vi "Display Module.vi"(7 "Callling VI":refnum<vi>) -> ()   [LabVIEW 2021]
uses:
  Display Module TypeDefs/IMAQ Z Scale Bar.ctl
  <vilib>/Utility/miscctls.llb/LVPointTypeDef.ctl
  <vilib>/vision/Image Controls.llb/IMAQ Image.ctl
  Hardware Configuration/Hardware Configuration Controls/Standard Action.ctl
  <vilib>/Utility/miscctls.llb/LVRectTypeDef.ctl
  <vilib>/event_ctls.llb/lveventtype.ctl
  Tools/TIFF Image Read and Write/ImageJ TIF Type Defs/TIF Write Image Information.ctl
  <vilib>/vision/NI_Vision_Development_Module.lvlib
panel:
  in  "Max":i32
  in  "Min":i32
  in  "lock scale":bool
  in  "Settings Menu":T1
  in  "Settings":bool
  in  "Refresh Rate (ms)":u32=30
  in  "Z Scale Channel 6":T2
  in  "Z Scale Channel 5":T2
  in  "Z Scale Channel 4":T2
  in  "Z Scale Channel 3":T2
  in  "Z Scale Channel 2":T2
  in  "Z Scale Channel 1":T2
  out "Messages":string
  in  "Max Left":bool
  in  "Max Right":bool
  in  "Add Display":bool
  in  "Remove Display":bool
  in  "Exit":bool
  out "Channel 6":T3(plugin-control)
  out "Channel 5":T3(plugin-control)
  out "Channel 4":T3(plugin-control)
  out "Channel 3":T3(plugin-control)
  out "Channel 2":T3(plugin-control)
  out "Channel 1":T3(plugin-control)
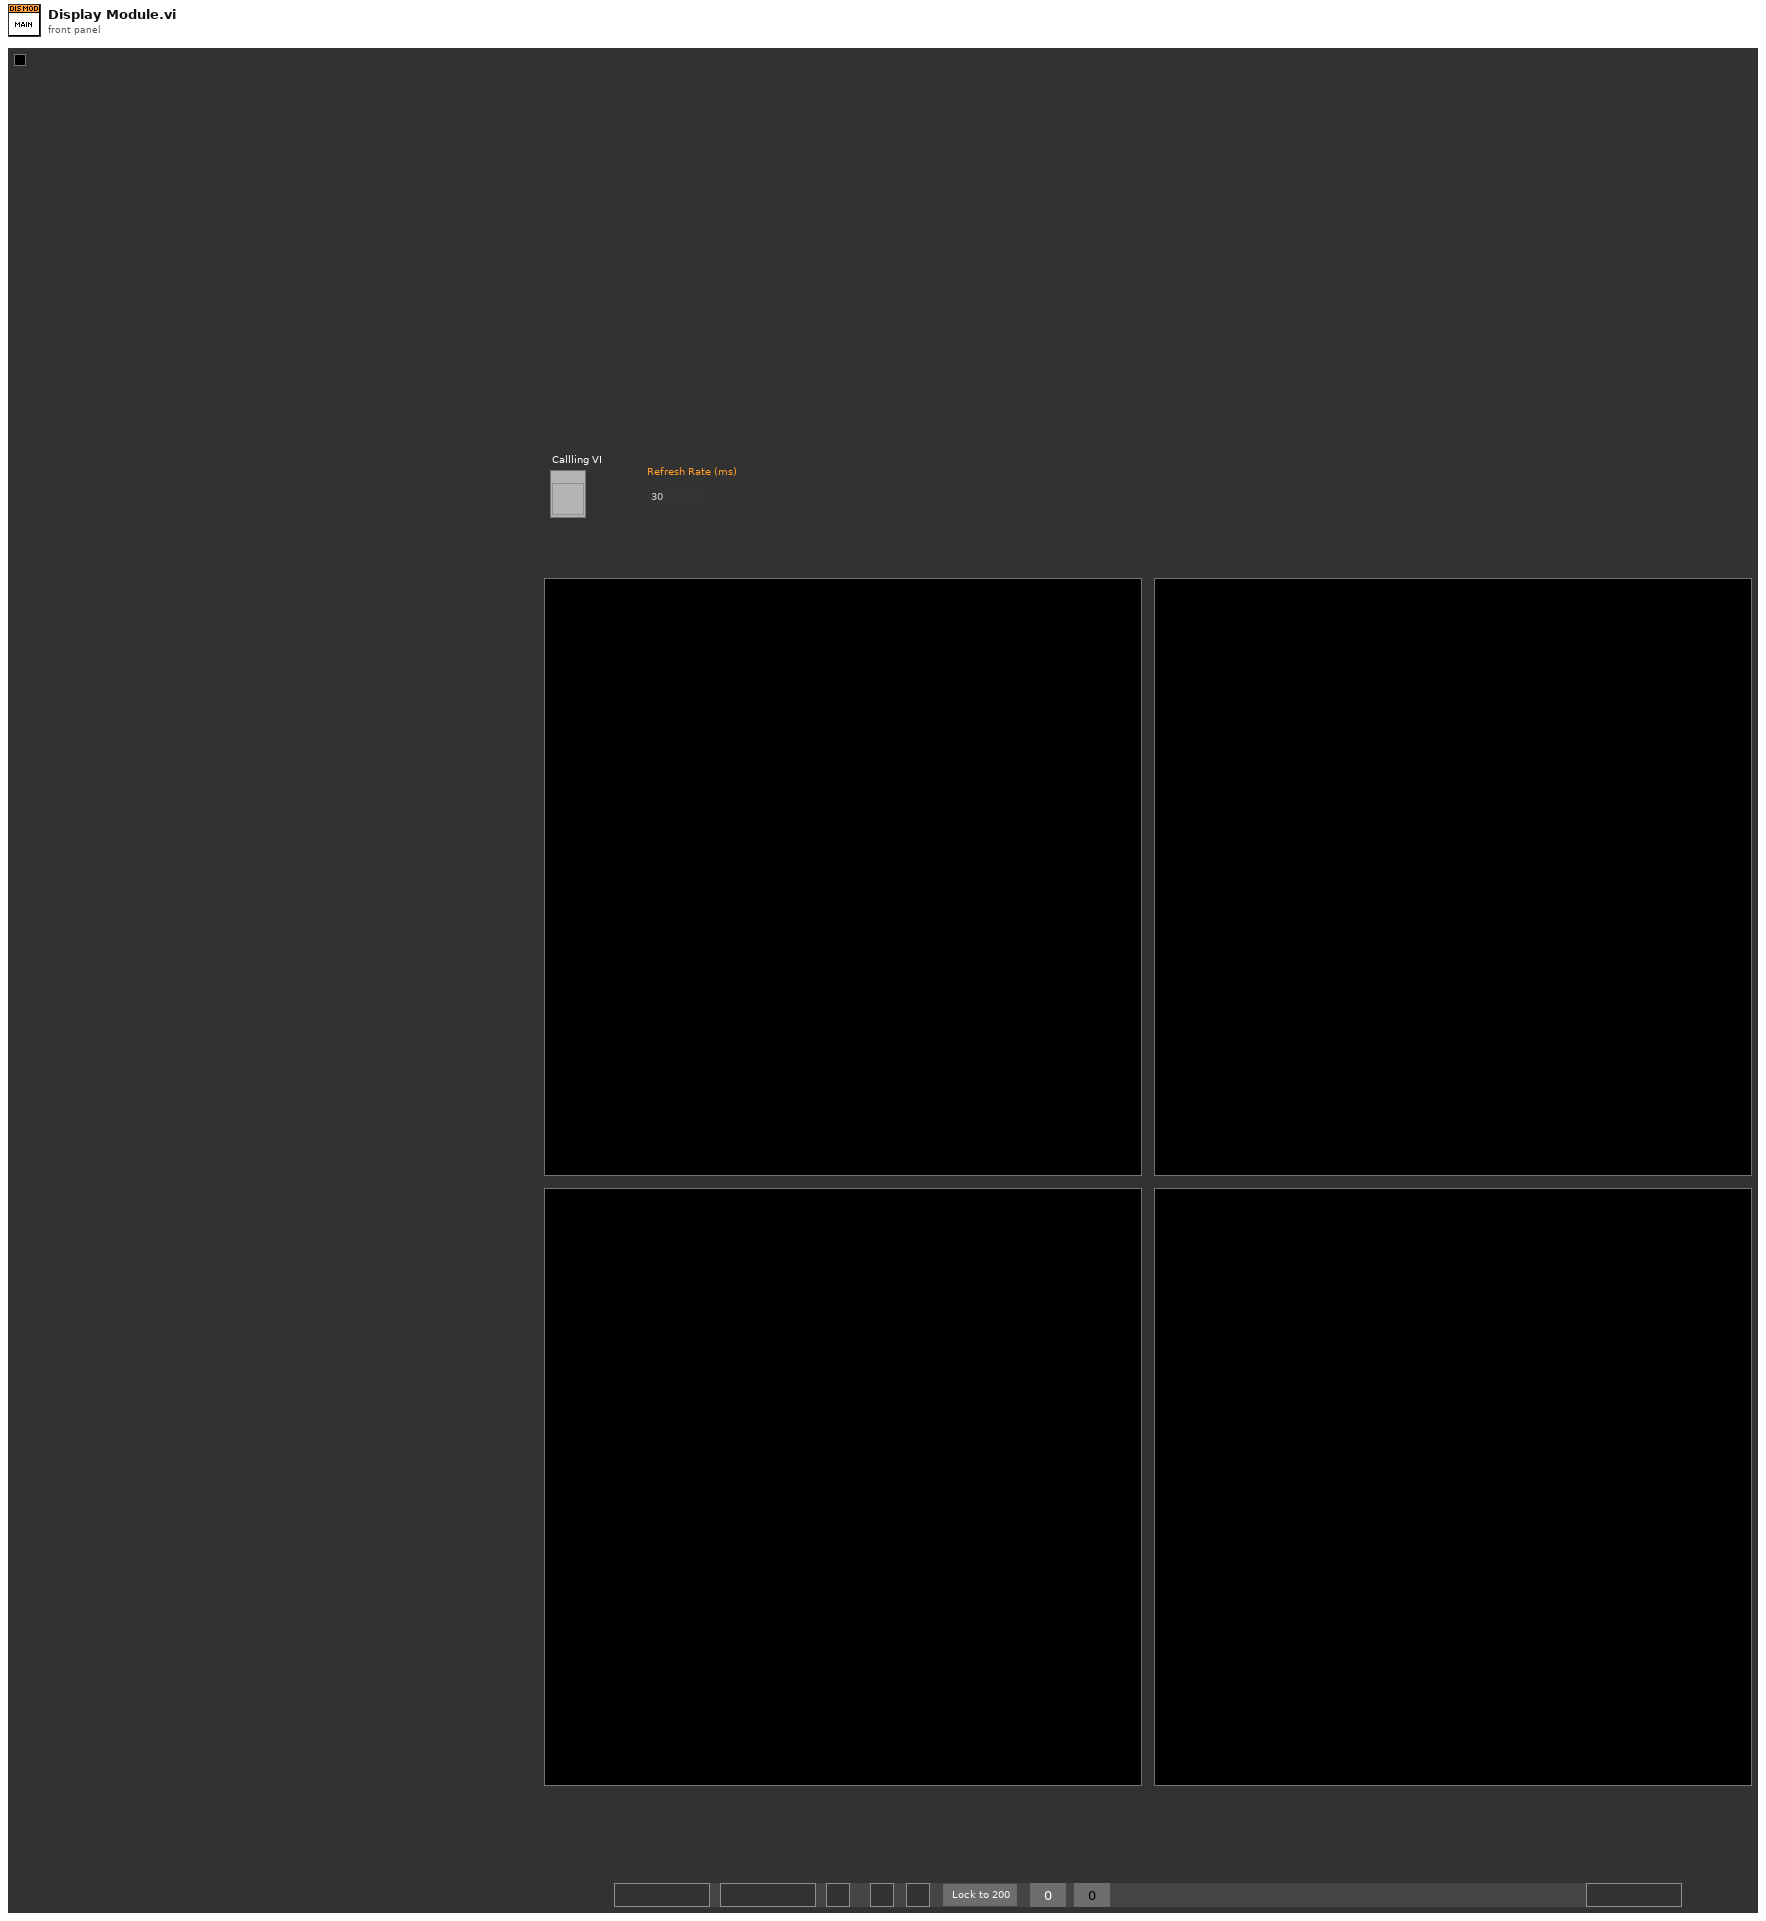
[diagram p1: front panel]
types:
  T1 = cluster{"Refresh Rate":bool, "Change Display Order":bool, "Display On / Off":bool}
  T2 = typedef "IMAQ Z Scale Bar.ctl" = cluster{"Z Scale Image":T3, "Z Scale Min":sgl, "Z Scale Max":sgl}
  T3 = typedef "IMAQ Image.ctl" = refnum<image>
  T4 = typedef "Standard Action.ctl" = enum16{"Read", "Write"}
  T5 = typedef "Image Type" = u32
  T6 = typedef "LVPointTypeDef.ctl" = cluster{"Horizontal":i16, "Vertical":i16}
  T7 = enum32{"Invalid", "Standard", "Closed", "Hidden", "Minimized", "Maximized"}
  T8 = enum16{"Always On", "Always Off", "Off While Running"}
  T9 = enum16{"Change Number", "Refresh Positions", "Get No. of Displays"}
  T10 = typedef "LVRectTypeDef.ctl" = cluster{"Left":i16, "Top":i16, "Right":i16, "Bottom":i16}
  T11 = typedef "lveventtype.ctl" = enum32{"Null", "Timeout", "Annotation Menu Selection", "Annotation Menu Selection?", "App Instance Close", "App Instance Close?", "Autoscale Range Change", "Bookmark Info Change", "Cell Edit", "Cell Edit?", "Cursor Grab", "Cursor Grab?", "Cursor Menu Selection", "Cursor Menu Selection?", "Cursor Move", "Cursor Release", "Data Change", "Direction Change", "Display State Change", "Drag Ended", "Drag Enter", "Drag Leave", "Drag Over", "Drag Source Update", "Drag Starting", "Drag Starting?", "Drop", "Exec State Change", "Key Down", "Key Down?", "Key Repeat", "Key Repeat?", "Key Up", "Listbox Double Click", "Menu Activation?", "Menu Selection (App)", "Menu Selection? (App)", "Menu Selection (User)", "Mouse Down", "Mouse Down?", "Mouse Enter", "Mouse Leave", "Mouse Move", "Mouse Up", "Mouse Wheel", "NI Security User Change (App)", "Pane Size", "Panel Close", "Panel Close?", "Panel Resize", "Plot Attribute Change", "Scale Range Change", "Shortcut Menu Activation?", "Shortcut Menu Selection (App)", "Shortcut Menu Selection? (App)", "Shortcut Menu Selection (User)", "Tree Double Click", "Tree Drag", "Tree Drag?", "Tree Drop", "Tree Drop?", "Tree Item Close", "Tree Item Close?", "Tree Item Open", "Tree Item Open?", "User Event", "Value Change"}
  T12 = cluster{"Global Rectangle":i32[], "Contours":cluster{"Contour Type":u32, "ROI Type":u32, "Points":i32[]}[]}
  T13 = cluster{"Mean Value":sgl, "Standard Variation":sgl, "Minimal Value":sgl, "Maximal Value":sgl, "Area (calibrated)":sgl, "Area (pixels)":u32, "%":sgl, "Calibration Valid":bool}
  T14 = typedef "TIF Write Image Information.ctl" = cluster{"Image Width (Pixels)":u32, "Image Height (Pixels)":u32, "Pixel Width (µm)":dbl, "Pixel Height (µm)":dbl, "Bits Per Sample (e.g. 16)":u32, "No. of Frames":u32, "No. of Slices":u32, "Time Step (sec)":dbl, "Z Step (µm)":dbl}
  T15 = typedef "LVAllMonitorsDisplayTypeDef.ctl" = cluster{"Bounds":cluster{"Left":i16, "Top":i16, "Right":i16, "Bottom":i16}, "Depth":i16}[]
  T16 = cluster{"Bounds":cluster{"Left":i16, "Top":i16, "Right":i16, "Bottom":i16}, "Depth":i16}
  T17 = enum16{"big-endian, network order", "native, host order", "little-endian"}
  T18 = cluster{"Contour Type":u32, "ROI Type":u32, "Points":i32[]}[]
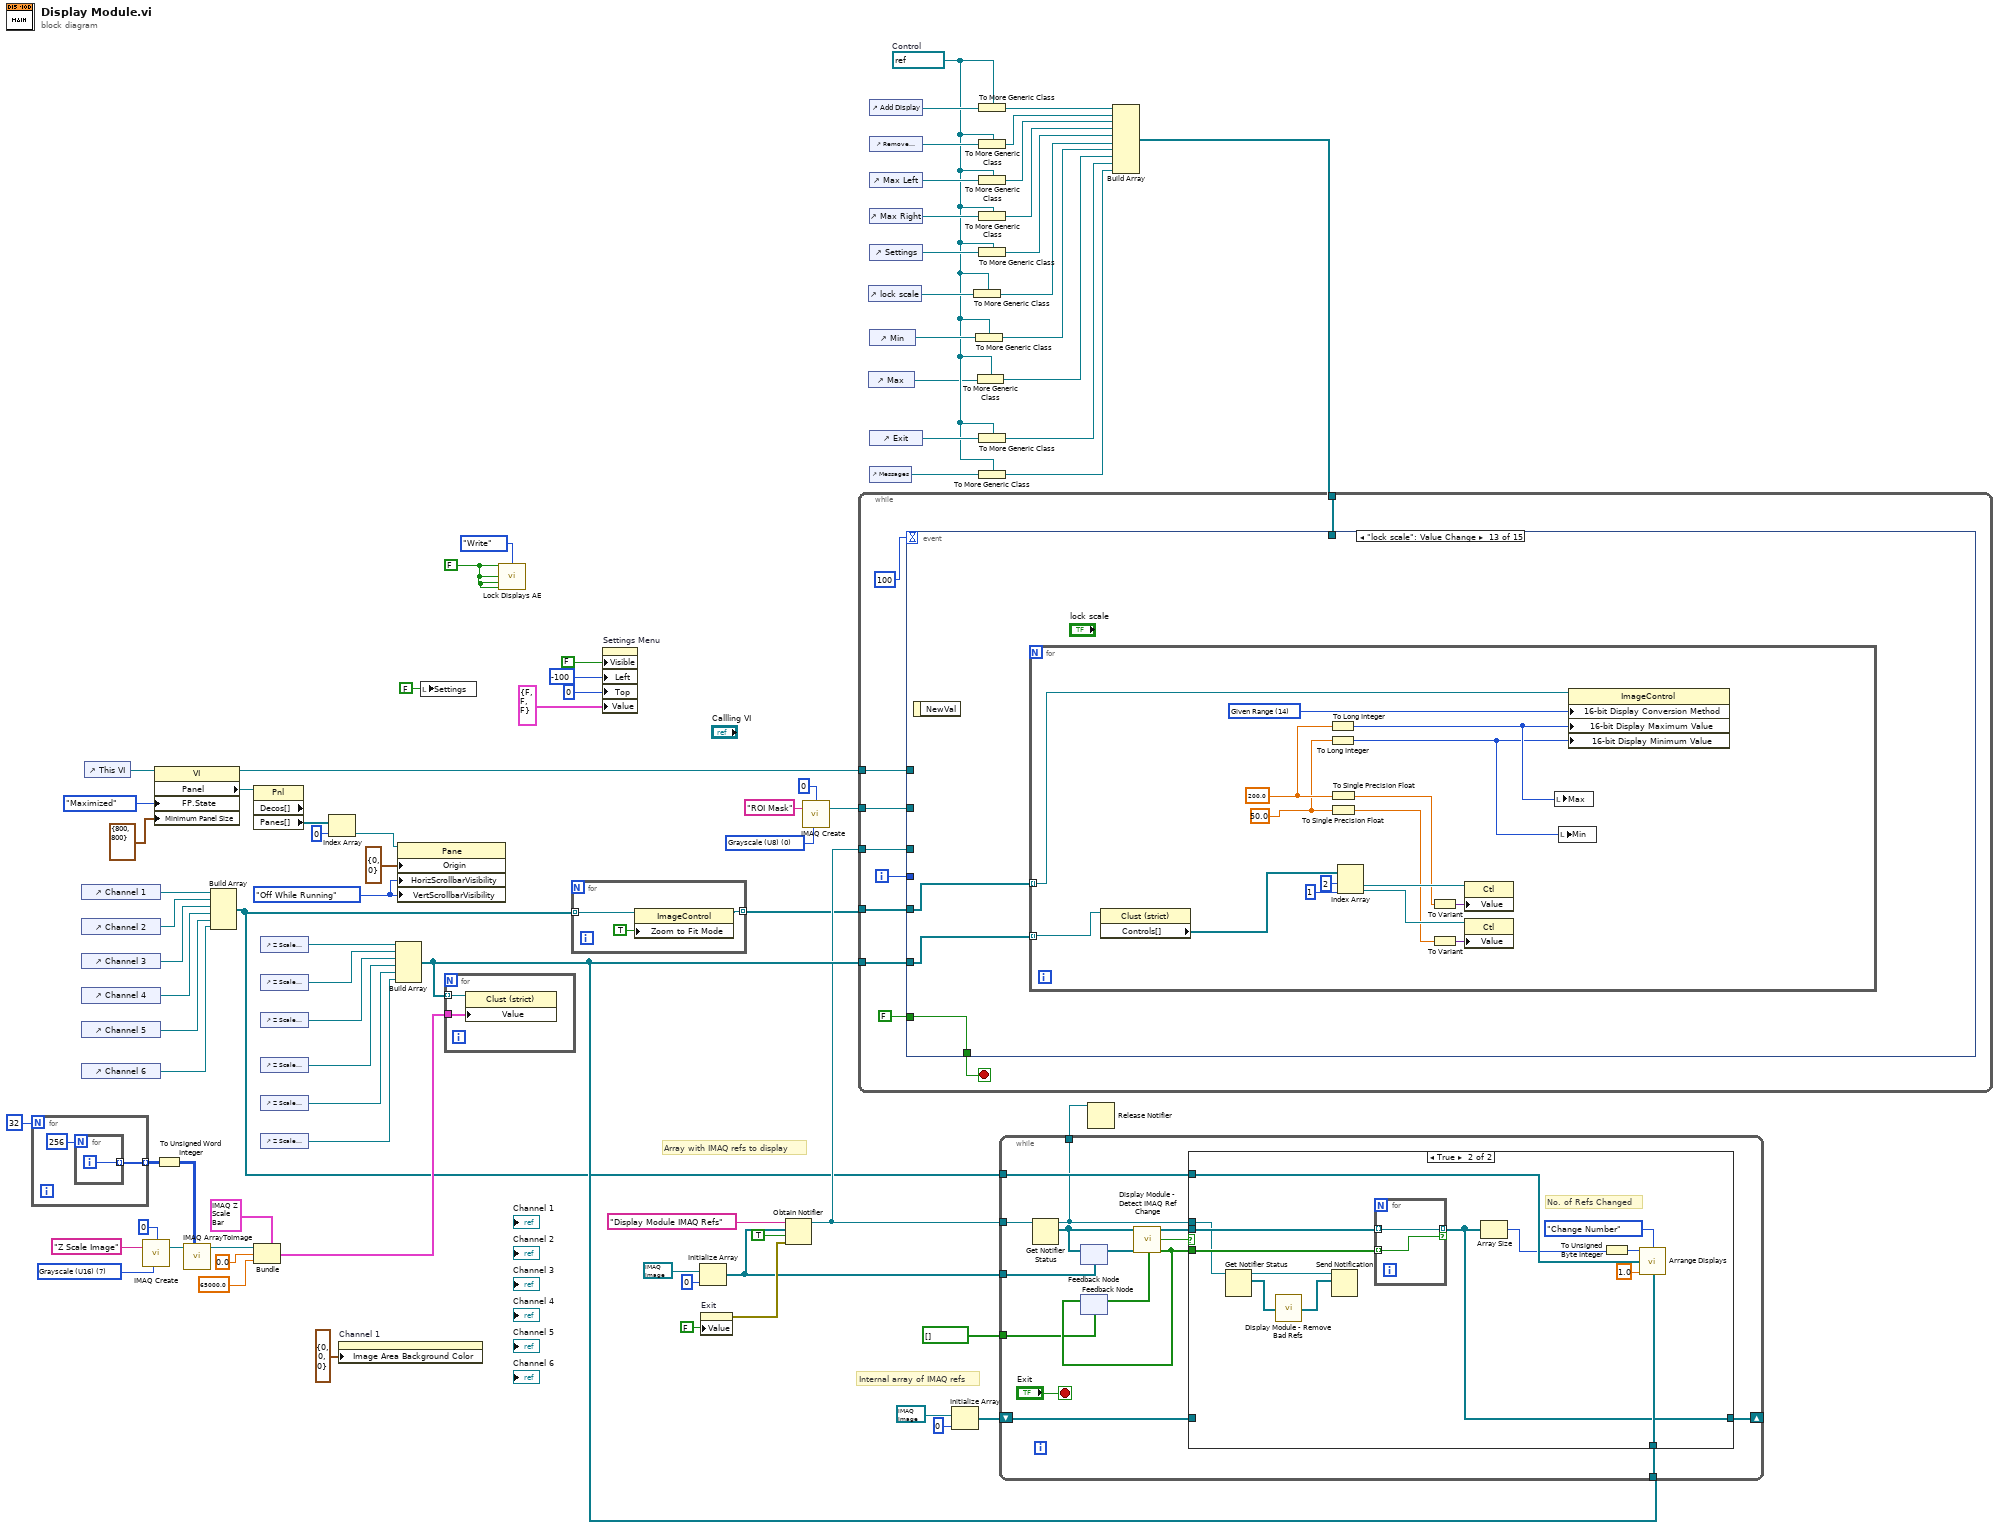
[diagram p0: block diagram]
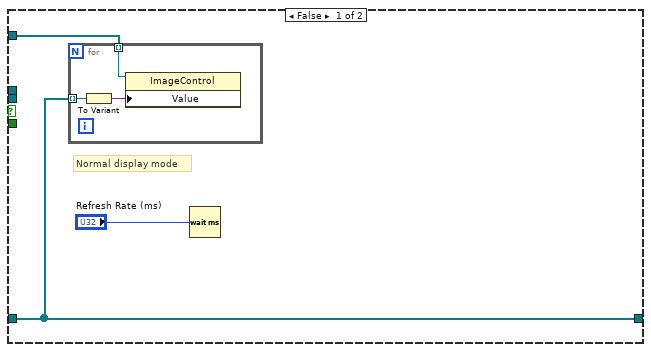
[diagram p2: hidden frame]
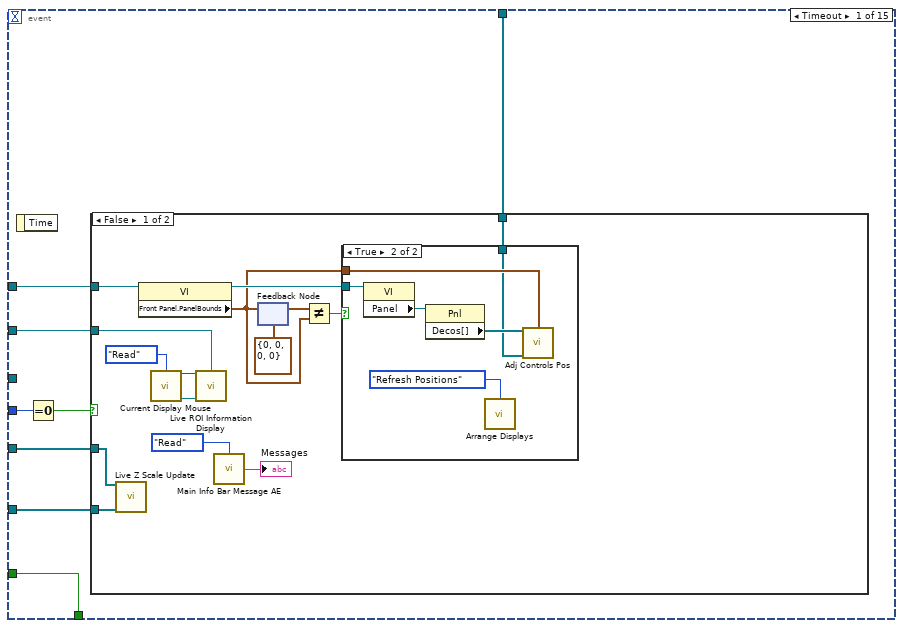
[diagram p3: hidden frame]
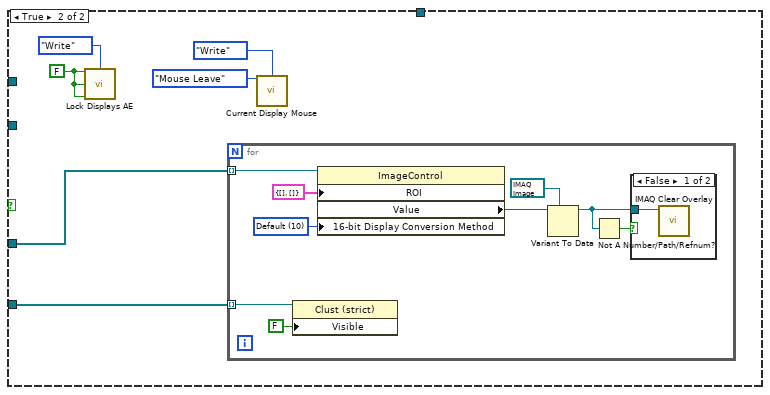
[diagram p5: hidden frame]
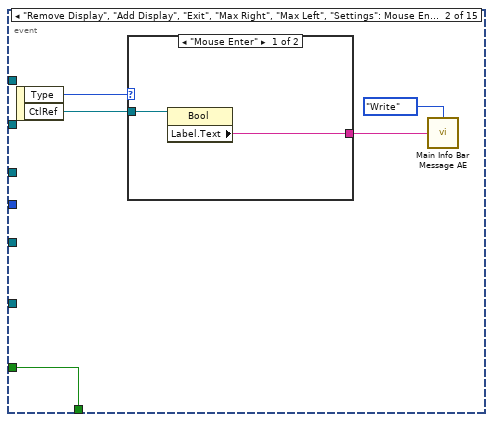
[diagram p7: hidden frame]
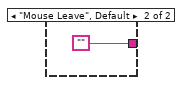
[diagram p8: hidden frame]
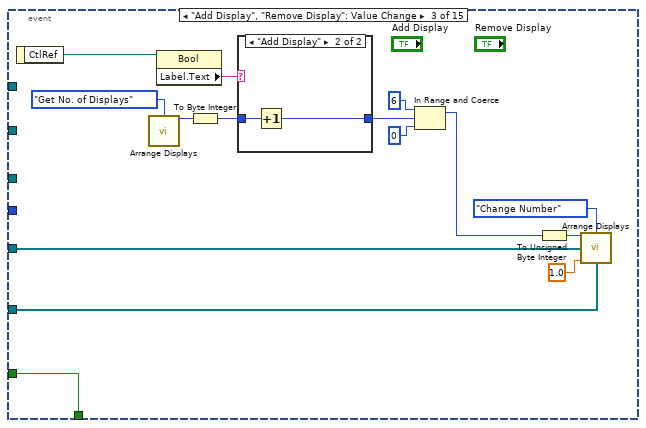
[diagram p9: hidden frame]
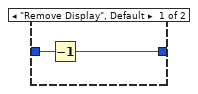
[diagram p10: hidden frame]
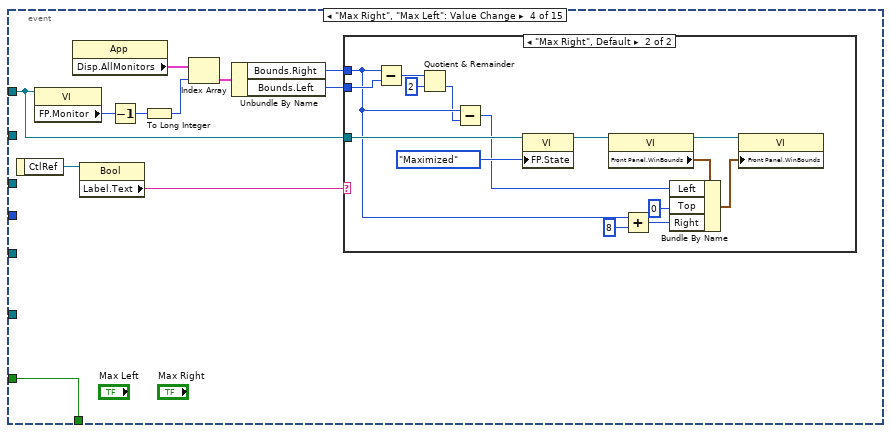
[diagram p11: hidden frame]
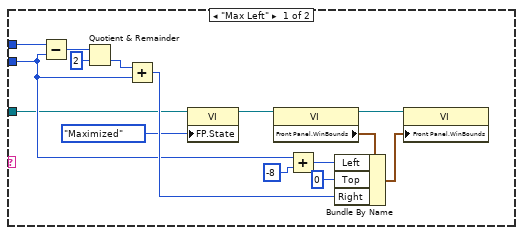
[diagram p12: hidden frame]
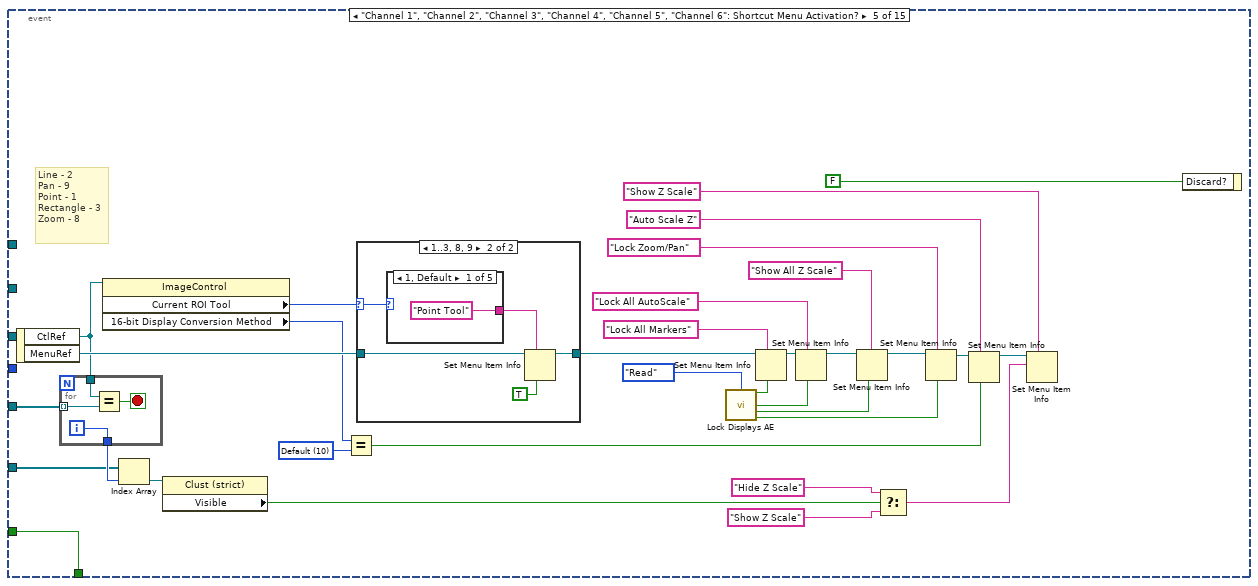
[diagram p13: hidden frame]
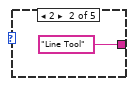
[diagram p15: hidden frame]
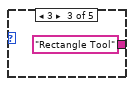
[diagram p16: hidden frame]
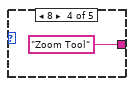
[diagram p17: hidden frame]
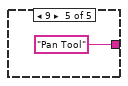
[diagram p18: hidden frame]
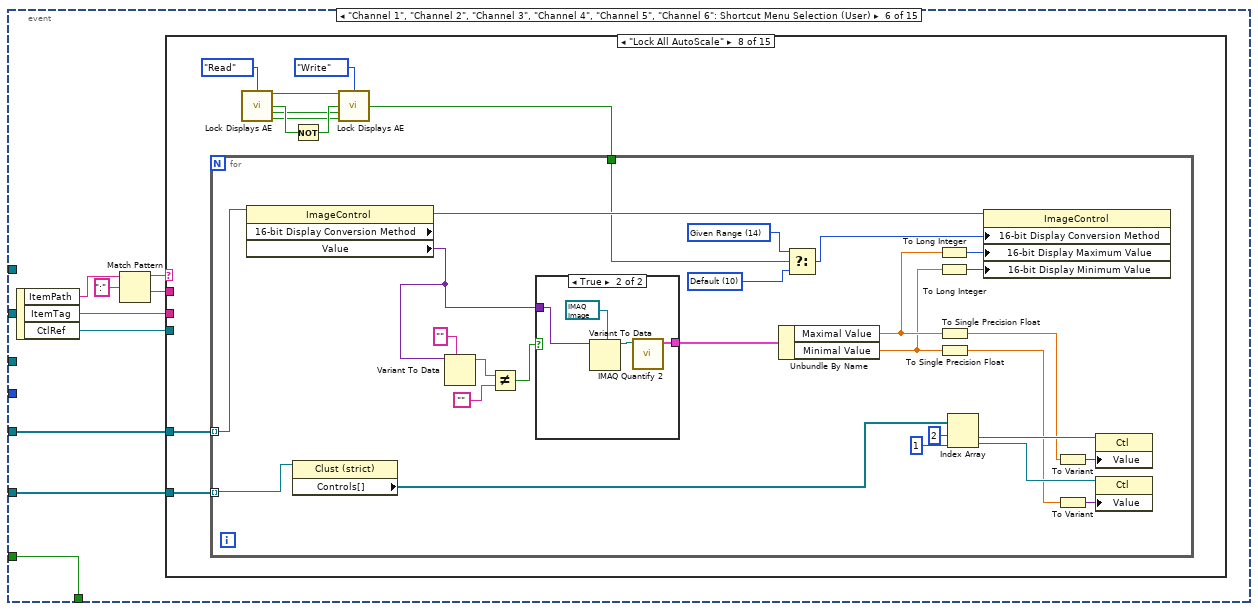
[diagram p19: hidden frame]
diagram:
  w12 = FALSE ("Lock All Markers")
  w3 = refnum<vi> refnum  # Control
  w56 = T5 7 items=["Grayscale (U8)", "Grayscale (I16)", "Grayscale (SGL)", "Complex (CSG)", "RGB (U32)", "HSL (U32)", "RGB (U64)", "Grayscale (U16)"] ("Image Type")
  w62 = T5 0 items=["Grayscale (U8)", "Grayscale (I16)", "Grayscale (SGL)", "Complex (CSG)", "RGB (U32)", "HSL (U32)", "RGB (U64)", "Grayscale (U16)"] ("Image Type")
  w75 = T8."Off While Running" ("Vertical Scrollbar Visibility")
  # "Internal array of IMAQ refs"
  # "Array with IMAQ refs to display"
  n1 = for {
    N: 32 -> [_]
    tunnel: [w85] -> w54 mode=indexing
    n2 = for {
      N: 256 -> [_]
      tunnel: [w87] -> w85 mode=indexing
      i -> [w87]
    }
  }
  n3 = control-ref of="Channel 1"() -> (w84:refnum<vi>)
  n4 = control-ref of="Channel 2"() -> (w79:refnum<vi>)
  n5 = control-ref of="Channel 3"() -> (w80:refnum<vi>)
  n6 = control-ref of="Channel 4"() -> (w81:refnum<vi>)
  n7 = control-ref of="Channel 5"() -> (w82:refnum<vi>)
  n8 = control-ref of="Channel 6"() -> (w83:refnum<vi>)
  n9 = control-ref of="This VI"() -> (w74:refnum<vi>)
  n10 = call "IMAQ Create"("Border Size"=0, "Image Name"="Z Scale Image", "Image Type"=w56) -> ("New Image"=w55:T3)  [unwired: 2 in, 1 out]
  n11 = property class="VI"(reference=w74, "FP.State"=T7."Maximized" ("Front Panel Window:State"), "Minimum Panel Size"=T6 {"Horizontal"=800, "Vertical"=800} ("Front Panel Window:Minimum Size")) -> (reference out=w69:refnum<vi>, "Panel"=w70:refnum<vi>)  [unwired: 1 in, 1 out]
  n12 = To Unsigned Word Integer(number=w54) -> (unsigned 16bit integer=w53:u16[][])
  n13 = call "IMAQ ArrayToImage"("Image Pixels (U16)"=w53, "Image"=w55) -> ("Image Out"=w52:T3)  [unwired: 8 in, 1 out]
  n14 = Build Array(w84, w79, w80, w81, w82, w83) -> (w11:refnum<vi>[])
  n15 = property class="Pnl" props=["Decos[]", "Panes[]"](reference=w70) -> ("Panes[]"=w71:refnum<vi>[])  [unwired: 1 in, 3 out]
  n16 = Bundle(cluster=T2 {"Z Scale Image"="remote image 00000232D697A428", "Z Scale Min"=0.0, "Z Scale Max"=65000.0} ("Z Scale Channel 6"), "Z Scale Image"=w52, "Z Scale Min"=sgl 0.0, "Z Scale Max"=sgl 65000.0) -> (w43:T2)
  n17 = control-ref of="Z Scale Channel 1"() -> (w49:refnum<vi>)
  n18 = control-ref of="Z Scale Channel 2"() -> (w44:refnum<vi>)
  n19 = control-ref of="Z Scale Channel 3"() -> (w45:refnum<vi>)
  n20 = control-ref of="Z Scale Channel 4"() -> (w46:refnum<vi>)
  n21 = control-ref of="Z Scale Channel 5"() -> (w47:refnum<vi>)
  n22 = control-ref of="Z Scale Channel 6"() -> (w48:refnum<vi>)
  n23 = Index Array(array=w71, index=0) -> (element=w77:refnum<vi>)
  n24 = property on="Channel 1" class="ImageControl"("Image Area Background Color"=cluster{"Red":u8, "Green":u8, "Blue":u8} {"Red"=0, "Green"=0, "Blue"=0} ("Image Area:Background:Background Color")) -> ()  [unwired: 2 in, 2 out]
  n25 = Build Array(w49, w44, w45, w46, w47, w48) -> (w41:refnum<vi>[])
  n26 = property class="Pane"(reference=w77, "Origin"=T6 {"Horizontal"=0, "Vertical"=0}, "HorizScrollbarVisibility"=w75, "VertScrollbarVisibility"=w75) -> ()  [unwired: 1 in, 2 out]
  n27 = local write "Settings"(FALSE ("Settings")) -> ()
  n28 = for {
    tunnel: w41 -> [w89] mode=indexing
    tunnel: w43 -> [w88]
    n29 = property class="Clust (strict)"(reference=w89, "Value"=w88) -> ()  [unwired: 1 in, 2 out]
  }
  n30 = call "Lock Displays AE.vi"("Lock All Markers"=w12, "Action"=Standard_Action."Write", "Lock All AutoScale"=w12, "Show All Z Scale"=w12, "Lock Pan/Zoom"=w12) -> ()  [unwired: 7 in, 4 out]
  n31 = for {
    tunnel: w11 -> [w92] mode=indexing
    tunnel: [w90] -> w10 mode=indexing
    n32 = property class="ImageControl"(reference=w92, "Zoom to Fit Mode"=TRUE) -> (reference out=w90:refnum<vi>)  [unwired: 1 in, 1 out]
  }
  n33 = property on="Settings Menu" class="Clust (strict)"("Visible"=FALSE, "Left"=-100 ("Position:Left"), "Top"=0 ("Position:Top"), "Value"=T1 {"Refresh Rate"=FALSE, "Change Display Order"=FALSE, "Display On / Off"=FALSE} ("Settings Menu")) -> ()  [unwired: 2 in, 2 out]
  n34 = Initialize Array(T3 refnum ("New Image"), 0 ("dimension size")) -> (w16:T3[])
  n35 = property on="Exit" class="Bool (strict)"("Value"=FALSE ("Exit")) -> (error out=w38:errorcluster)  [unwired: 2 in, 1 out]
  n36 = Obtain Notifier(name (unnamed)="Display Module IMAQ Refs", notification data type=w16, create if not found? (T)=TRUE, error in (no error)=w38) -> (notifier out=w15:refnum<notifier>)  [unwired: 2 out]
  n37 = call "IMAQ Create"("Border Size"=0, "Image Name"="ROI Mask", "Image Type"=w62) -> ("New Image"=w60:T3)  [unwired: 2 in, 1 out]
  n38 = control-ref of="lock scale"() -> (w9:refnum<vi>)
  n39 = control-ref of="Max"() -> (w2:refnum<vi>)
  n40 = control-ref of="Add Display"() -> (w37:refnum<vi>)
  n41 = control-ref of="Remove Display"() -> (w31:refnum<vi>)
  n42 = control-ref of="Max Left"() -> (w32:refnum<vi>)
  n43 = control-ref of="Max Right"() -> (w33:refnum<vi>)
  n44 = control-ref of="Settings"() -> (w34:refnum<vi>)
  n45 = control-ref of="Min"() -> (w7:refnum<vi>)
  n46 = control-ref of="Exit"() -> (w35:refnum<vi>)
  n47 = control-ref of="Messages"() -> (w36:refnum<vi>)
  n48 = Initialize Array(T3 refnum ("New Image"), 0 ("dimension size")) -> (w17:T3[])
  n49 = To More Generic Class(target class=w3, reference=w9) -> (generic class reference=w8:refnum<vi>)
  n50 = To More Generic Class(target class=w3, reference=w7) -> (generic class reference=w4:refnum<vi>)
  n51 = To More Generic Class(target class=w3, reference=w2) -> (generic class reference=w1:refnum<vi>)
  n52 = To More Generic Class(target class=w3, reference=w37) -> (generic class reference=w30:refnum<vi>)
  n53 = To More Generic Class(target class=w3, reference=w31) -> (generic class reference=w29:refnum<vi>)
  n54 = To More Generic Class(target class=w3, reference=w32) -> (generic class reference=w28:refnum<vi>)
  n55 = To More Generic Class(target class=w3, reference=w33) -> (generic class reference=w27:refnum<vi>)
  n56 = To More Generic Class(target class=w3, reference=w34) -> (generic class reference=w26:refnum<vi>)
  n57 = To More Generic Class(target class=w3, reference=w35) -> (generic class reference=w5:refnum<vi>)
  n58 = To More Generic Class(target class=w3, reference=w36) -> (generic class reference=w6:refnum<vi>)
  n59 = while {
    tunnel: w15 -> [w107]
    tunnel: w11 -> [w106]
    tunnel: [w96] -> w64
    tunnel: w41 -> [w104]
    shift-right: [w97] -> _
    shift-left: w17 -> [w103]
    tunnel: w16 -> [w100]
    tunnel: bool[] [] -> [w93]
    stop <- "Exit" stop-if-true
    n60 = Get Notifier Status(notifier=w107) -> (notifier out=w96:refnum<notifier>, current notification=w102:T3[])  [unwired: 1 in, 3 out]
    n61 = feedback-in #1(w102) -> ()
    n62 = feedback #1(w100) -> (w101:T3[])
    n63 = feedback #2(w93) -> (w94:bool[])
    n64 = call "Display Module - Detect IMAQ Ref Change.vi"("Current Image Refs"=w102, "Previous Image Refs"=w101, "Previous Image Display Flags"=w94) -> ("Current Image Refs (Dup)"=w99:T3[], "Change Detected"=w98:bool, "Image Display Flags"=w95:bool[])  [unwired: 10 in]
    n65 = feedback-in #2(w95) -> ()
    n66 = case shown="True" w98 {
      tunnel: w99 -> [_ w121]
      tunnel: w106 -> [w110 w123]
      tunnel: w104 -> [_ w124]
      tunnel: w103 -> [w108 _]
      tunnel: w95 -> [_ w120]
      tunnel: [w108 w118] -> w97
      tunnel: w96 -> [_ w114]
      frame False {
        # "Normal display mode"
        n67 = for {
          tunnel: w110 -> [w113] mode=indexing
          tunnel: w108 -> [w111] mode=indexing
          n68 = To Variant(anything=w111) -> (Variant=w112:variant)
          n69 = property class="ImageControl"(reference=w113, "Value"=w112) -> ()  [unwired: 1 in, 2 out]
        }
        n70 = Wait (ms)(milliseconds to wait="Refresh Rate (ms)") -> ()  [unwired: 1 out]
      }
      frame True {
        # "No. of Refs Changed"
        n71 = Get Notifier Status(notifier=w114) -> (notifier out=w116:refnum<notifier>, current notification=w115:T3[])  [unwired: 1 in, 3 out]
        n72 = call "Display Module - Remove Bad Refs.vi"("Image Refs In"=w115) -> ("Image Refs Out"=w117:T3[])  [unwired: 14 in]
        n73 = Send Notification(notification=w117, notifier=w116) -> ()  [unwired: 1 in, 2 out]
        n74 = for {
          tunnel: w121 -> [w128] mode=indexing
          tunnel: [w128] -> w118 mode=indexing if=w127
          tunnel: w120 -> [w127] mode=indexing
        }
        n75 = Array Size(array=w118) -> (size(s)=w119:i32)
        n76 = To Unsigned Byte Integer(number=w119) -> (unsigned 8bit integer=w126:u8)
        n77 = call "Arrange Displays.vi"("Number of Displays"=w126, "Action"=T9."Change Number", "IMAQ Display Refs"=w123, "Aspect Ratio (Width/Height)"=1.0, "Z Scale Refs"=w124) -> ()  [unwired: 9 in, 2 out]
      }
    }
  }
  n78 = Release Notifier(notifier=w64) -> ()  [unwired: 2 in, 3 out]
  n79 = Build Array(w30, w29, w28, w27, w26, w8, w4, w1, w5, w6) -> (w25:refnum<vi>[])
  n80 = while {
    tunnel: w10 -> [w137]
    tunnel: w69 -> [w133]
    tunnel: w60 -> [w132]
    tunnel: w41 -> [w131]
    tunnel: w25 -> [w130]
    tunnel: w15 -> [w129]
    i -> [w138]
    stop <- w136 stop-if-true
    n81 = event shown="[12] \"lock scale\": Value Change" {
      selector: _ -> [_ _ _ _ _ _ _ _ _ _ _ _ _ _ _]
      dyn-events: _ -> [_ _ _ _ _ _ _ _ _ _ _ _ _ _ _]
      timeout: 100 -> [_ _ _ _ _ _ _ _ _ _ _ _ _ _ _]
      tunnel: w138 -> [w146 _ _ _ _ _ _ _ _ _ _ _ _ _ _]
      tunnel: w137 -> [w144 _ w193 _ w260 w302 w553 _ w589 w597 _ w624 w659 w678 w696]
      tunnel: [w143 w188 w206 w221 w283 w308 w558 w580 w591 w603 w613 w636 w657 w676 w697] -> w136
      tunnel: FALSE -> [w143 w188 w206 w221 w283 w308 w558 w580 w591 w603 w613 w636 w657 w676 _]
      tunnel: w133 -> [w142 _ _ w212 _ _ _ _ _ _ _ _ _ _ _]
      tunnel: w132 -> [w141 _ _ _ _ _ _ _ _ _ _ _ _ _ w695]
      tunnel: w131 -> [w140 _ w194 _ w261 w301 _ _ w590 _ _ _ w658 w677 _]
      tunnel: w130 -> [w139 _ _ _ _ _ _ _ _ _ _ _ _ _ _]
      tunnel: w129 -> [_ _ _ _ _ _ _ _ _ _ _ w625 _ _ _]
      event Timeout {
        n82 = event-data() -> ()  [unwired: 1 in, 1 out]
        n83 = Equal To 0?(x=w146) -> (x = 0?=w145:bool)
        n84 = case shown="False" w145 {
          tunnel: w144 -> [w149 w171]
          tunnel: w142 -> [w161 _]
          tunnel: w141 -> [w155 _]
          tunnel: w140 -> [w148 w170]
          tunnel: w139 -> [w147 _]
          frame False {
            n85 = call "Live Z Scale Update.vi"("IMAQ Display Refs"=w149, "Z Scale Refs"=w148) -> ()  [unwired: 14 in]
            n86 = property class="VI"(reference=w161) -> (reference out=w157:refnum<vi>, "Front Panel.PanelBounds"=w156:T10)  [unwired: 1 in, 1 out]
            n87 = call "Current Display Mouse.vi"("Action"=Standard_Action."Read") -> ("Event Type Out"=w153:T11, "IMAQ Image Display Ref Out"=w152:refnum<vi>)  [unwired: 13 in]
            n88 = call "Live ROI Information Display.vi"("Event Type"=w153, "ROI Mask REF"=w155, "IMAQ Image Display Ref"=w152) -> ()  [unwired: 13 in]
            n89 = call "Main Info Bar Message AE.vi"("Action"=Standard_Action."Read") -> ("Message Out"=→"Messages":string)  [unwired: 14 in]
            n90 = feedback-in #3(w156) -> ()
            n91 = feedback #3(T10 {"Left"=0, "Top"=0, "Right"=0, "Bottom"=0} ("Front Panel.PanelBounds")) -> (w160:T10)
            n92 = Not Equal?(x=w160, y=w156) -> (x != y?=w158:bool)
            n93 = case shown="True" w158 {
              tunnel: w157 -> [_ w165]
              tunnel: w156 -> [_ w164]
              tunnel: w147 -> [_ w163]
              frame False {
              }
              frame True {
                n94 = property class="VI"(reference=w165) -> ("Panel"=w167:refnum<vi>)  [unwired: 1 in, 2 out]
                n95 = property class="Pnl"(reference=w167) -> ("Decos[]"=w166:refnum<vi>[])  [unwired: 1 in, 2 out]
                n96 = call "Arrange Displays.vi"("Action"=T9."Refresh Positions") -> ()  [unwired: 13 in, 2 out]
                n97 = call "Adj Controls Pos.vi"("Decoration Ref Array"=w166, "Panel Bounds"=w164, "Control Ref Array"=w163) -> ()  [unwired: 13 in]
              }
            }
          }
          frame True {
            w173 = FALSE ("Lock All Markers")
            n98 = call "Lock Displays AE.vi"("Lock All Markers"=w173, "Action"=Standard_Action."Write", "Lock All AutoScale"=w173, "Lock Pan/Zoom"=w173) -> ()  [unwired: 8 in, 4 out]
            n99 = for {
              tunnel: w171 -> [w177] mode=indexing
              tunnel: w170 -> [w176] mode=indexing
              w174 = u32 10 items=["Default"=10, "Most Significant Bits"=11, "Full Dynamic"=12, "Downshift"=13, "Given Range"=14, "90% Dynamic"=15, "Given Percent Range"=16] ("16-bit Display Mapping:Conversion Method")
              n100 = property class="Clust (strict)"(reference=w176, "Visible"=FALSE) -> ()  [unwired: 1 in, 2 out]
              n101 = property class="ImageControl"(reference=w177, "ROI"=T12 {"Global Rectangle"=[], "Contours"=[]}, "16-bit Display Conversion Method"=w174) -> ("Value"=w178:variant)  [unwired: 1 in, 2 out]
              n102 = Variant To Data(type=T3 refnum ("New Image"), Variant=w178) -> (data=w181:T3)  [unwired: 1 in, 1 out]
              n103 = Not A Number/Path/Refnum?(number/path/refnum=w181) -> (NaN/Path/Refnum?=w180:bool)
              n104 = case shown="False" w180 {
                tunnel: w181 -> [w183 _]
                frame False {
                  n105 = call "IMAQ Clear Overlay"("Image"=w183) -> ()  [unwired: 9 in, 2 out]
                }
                frame True {
                }
              }
            }
            n106 = call "Current Display Mouse.vi"("Event Type"=lveventtype."Mouse Leave", "Action"=Standard_Action."Write") -> ()  [unwired: 12 in, 2 out]
          }
        }
      }
      event "Remove Display", "Add Display", "Exit", "Max Right", "Max Left", "Settings", "Settings Menu.Refresh Rate", "Settings Menu.Change Display Order", "Settings Menu.Display On / Off": Mouse Enter; "Remove Display", "Add Display", "Exit", "Max Right", "Max Left", "Settings", "Settings Menu.Refresh Rate", "Settings Menu.Change Display Order", "Settings Menu.Display On / Off": Mouse Leave {
        n107 = event-data() -> ("Type"=w187:T11, "CtlRef"=w186:refnum<vi>)  [unwired: 1 in]
        n108 = case shown="\"Mouse Enter\"" w187 {
          tunnel: w186 -> [w190 _]
          tunnel: [w189 ""] -> w184
          frame "Mouse Enter" {
            n109 = property class="Bool"(reference=w190) -> ("Label.Text"=w189:string)  [unwired: 1 in, 2 out]
          }
          frame "Mouse Leave", Default {
          }
        }
        n110 = call "Main Info Bar Message AE.vi"("Action"=Standard_Action."Write", "Message"=w184) -> ()  [unwired: 13 in, 1 out]
      }
      event "Add Display", "Remove Display": Value Change {
        n111 = event-data() -> ("CtlRef"=w205:refnum<vi>)  [unwired: 1 in]
        n112 = call "Arrange Displays.vi"("Action"=T9."Get No. of Displays") -> ("Number of Displays Out"=w196:u8)  [unwired: 13 in, 1 out]
        n113 = property class="Bool"(reference=w205) -> ("Label.Text"=w204:string)  [unwired: 1 in, 2 out]
        n114 = To Byte Integer(number=w196) -> (8bit integer=w195:i8)
        n115 = case shown="\"Add Display\"" w204 {
          tunnel: w195 -> [w208 w210]
          tunnel: [w207 w209] -> w201
          frame "Remove Display", Default {
            n116 = Decrement(x=w208) -> (x-1=w207:i8)
          }
          frame "Add Display" {
            n117 = Increment(x=w210) -> (x+1=w209:i8)
          }
        }
        n118 = In Range and Coerce(upper limit=i8 6, x=w201, lower limit=i8 0) -> (coerced(x)=w200:i8)  [unwired: 1 out]
        n119 = To Unsigned Byte Integer(number=w200) -> (unsigned 8bit integer=w199:u8)
        n120 = call "Arrange Displays.vi"("Number of Displays"=w199, "Action"=T9."Change Number", "IMAQ Display Refs"=w193, "Aspect Ratio (Width/Height)"=1.0, "Z Scale Refs"=w194) -> ()  [unwired: 9 in, 2 out]
      }
      event "Max Right", "Max Left": Value Change {
        n121 = event-data() -> ("CtlRef"=w220:refnum<vi>)  [unwired: 1 in]
        n122 = property class="VI"(reference=w212) -> ("FP.Monitor"=w219:u16)  [unwired: 1 in, 2 out]
        n123 = property class="App"() -> ("Disp.AllMonitors"=w218:T15)  [unwired: 2 in, 2 out]
        n124 = property class="Bool"(reference=w220) -> ("Label.Text"=w211:string)  [unwired: 1 in, 2 out]
        n125 = Decrement(x=w219) -> (x-1=w217:u16)
        n126 = To Long Integer(number=w217) -> (32bit integer=w216:i32)
        n127 = Index Array(array=w218, index=w216) -> (element=w215:T16)
        n128 = Unbundle By Name(w215) -> ("Bounds.Right"=w214:i16, "Bounds.Left"=w213:i16)
        n129 = case shown="\"Max Right\", Default" w211 {
          tunnel: w214 -> [w236 w239]
          tunnel: w213 -> [w224 w243]
          tunnel: w212 -> [w222 w242]
          frame "Max Left" {
            n130 = Subtract(x=w236, y=w224) -> (x-y=w231:i16)
            n131 = Quotient & Remainder(x=w231, y=i16 2) -> (floor(x/y)=w229:i16)  [unwired: 1 out]
            n132 = Add(x=w229, y=w224) -> (x+y=w228:i16)
            n133 = property class="VI"(reference=w222, "FP.State"=T7."Maximized" ("Front Panel Window:State")) -> (reference out=w226:refnum<vi>)  [unwired: 1 in, 1 out]
            n134 = property class="VI"(reference=w226) -> (reference out=w235:refnum<vi>, "Front Panel.WinBounds"=w233:T10)  [unwired: 1 in, 1 out]
            n135 = Add(x=w224, y=i16 -8 ("Left")) -> (x+y=w223:i16)
            n136 = Bundle By Name(cluster=w233, "Left"=w223, "Top"=i16 0, "Right"=w228) -> (w234:T10)
            n137 = property class="VI"(reference=w235, "Front Panel.WinBounds"=w234) -> ()  [unwired: 1 in, 2 out]
          }
          frame "Max Right", Default {
            n138 = Subtract(x=w239, y=w243) -> (x-y=w248:i16)
            n139 = Quotient & Remainder(x=w248, y=i16 2) -> (floor(x/y)=w238:i16)  [unwired: 1 out]
            n140 = Subtract(x=w239, y=w238) -> (x-y=w237:i16)
            n141 = property class="VI"(reference=w242, "FP.State"=T7."Maximized" ("Front Panel Window:State")) -> (reference out=w245:refnum<vi>)  [unwired: 1 in, 1 out]
            n142 = property class="VI"(reference=w245) -> (reference out=w251:refnum<vi>, "Front Panel.WinBounds"=w249:T10)  [unwired: 1 in, 1 out]
            n143 = Add(x=w239, y=i16 8 ("Left")) -> (x+y=w240:i16)
            n144 = Bundle By Name(cluster=w249, "Left"=w237, "Top"=i16 0, "Right"=w240) -> (w250:T10)
            n145 = property class="VI"(reference=w251, "Front Panel.WinBounds"=w250) -> ()  [unwired: 1 in, 2 out]
          }
        }
      }
      event "Channel 1", "Channel 2", "Channel 3", "Channel 4", "Channel 5", "Channel 6": Shortcut Menu Activation? {
        w267 = u32 10 items=["Default"=10, "Most Significant Bits"=11, "Full Dynamic"=12, "Downshift"=13, "Given Range"=14, "90% Dynamic"=15, "Given Percent Range"=16] ("16-bit Display Mapping:Conversion Method")
        # "Line - 2\nPan - 9\nPoint - 1\nRectangle - 3\nZoom - 8"
        n146 = event-data() -> ("CtlRef"=w262:refnum<vi>, "MenuRef"=w281:refnum<k9>)  [unwired: 1 in]
        n147 = for {
          tunnel: w260 -> [w288] mode=indexing
          tunnel: w262 -> [w286]
          tunnel: [w285] -> w264
          i -> [w285]
          stop <- w287 stop-if-true
          n148 = Equal?(x=w286, y=w288) -> (x = y?=w287:bool)
        }
        n149 = property class="ImageControl"(reference=w262) -> ("Current ROI Tool"=w282:u32, "16-bit Display Conversion Method"=w269:u32)  [unwired: 1 in, 2 out]
        n150 = Index Array(array=w261, index=w264) -> (element=w263:refnum<vi>)
        n151 = property class="Clust (strict)"(reference=w263) -> ("Visible"=w256:bool)  [unwired: 1 in, 2 out]
        n152 = Equal?(x=w269, y=w267) -> (x = y?=w268:bool)
        n153 = case shown="1..3, 8, 9" w282 {
          selector: w282 -> [_ w294]
          tunnel: w281 -> [w289 w292]
          tunnel: [w289 w290] -> w280
          frame Default {
          }
          frame 1..3, 8, 9 {
            n154 = case shown="1, Default" w294 {
              tunnel: ["Point Tool" ("item tag") "Line Tool" ("item tag") "Rectangle Tool" ("item tag") "Zoom Tool" ("item tag") "Pan Tool" ("item tag")] -> w291
              frame 1, Default {
              }
              frame 2 {
              }
              frame 3 {
              }
              frame 8 {
              }
              frame 9 {
              }
            }
            n155 = Set Menu Item Info(6:TRUE ("checked"), 7:w291, 11:w292) -> (3:w290:refnum<k9>)  [unwired: 4 in, 1 out]
          }
        }
        n156 = call "Lock Displays AE.vi"("Action"=Standard_Action."Read") -> ("Lock All Markers Out"=w274:bool, "Lock All AutoScale Out"=w273:bool, "Show All Z Scale Out"=w252:bool, "Lock Pan/Zoom Out"=w272:bool)  [unwired: 11 in]
        n157 = Set Menu Item Info(6:w274, 7:"Lock All Markers" ("item tag"), 11:w280) -> (3:w279:refnum<k9>)  [unwired: 4 in, 1 out]
        n158 = Set Menu Item Info(6:w273, 7:"Lock All AutoScale" ("item tag"), 11:w279) -> (3:w255:refnum<k9>)  [unwired: 4 in, 1 out]
        n159 = Set Menu Item Info(6:w252, 7:"Show All Z Scale" ("item tag"), 11:w255) -> (3:w254:refnum<k9>)  [unwired: 4 in, 1 out]
        n160 = Select(t="Hide Z Scale" ("item tag"), s=w256, f="Show Z Scale" ("item tag")) -> (s? t:f=w257:string)
        n161 = Set Menu Item Info(6:w272, 7:"Lock Zoom/Pan" ("item tag"), 11:w254) -> (3:w271:refnum<k9>)  [unwired: 4 in, 1 out]
        n162 = Set Menu Item Info(6:w268, 7:"Auto Scale Z" ("item tag"), 11:w271) -> (3:w266:refnum<k9>)  [unwired: 4 in, 1 out]
        n163 = Set Menu Item Info(7:"Show Z Scale" ("item tag"), 10:w257, 11:w266) -> ()  [unwired: 4 in, 2 out]
        n164 = event-data("Discard?"=FALSE) -> ()  [unwired: 1 in, 1 out]
      }
      event "Channel 1", "Channel 2", "Channel 3", "Channel 4", "Channel 5", "Channel 6": Shortcut Menu Selection (User) {
        n165 = event-data() -> ("ItemPath"=w306:string, "ItemTag"=w307:string, "CtlRef"=w303:refnum<vi>)  [unwired: 1 in]
        n166 = Match Pattern(string=w306, regular expression=":") -> (before substring=w304:string, after substring=w300:string)  [unwired: 1 in, 2 out]
        n167 = case shown="\"Lock All AutoScale\"" w304 {
          selector: w304 -> [_ _ w341 _ _ _ _ _ _ _ w488 _ _ _ _]
          tunnel: w303 -> [_ w321 w347 w372 _ w394 _ _ w458 w469 w486 w510 _ _ w519]
          tunnel: w307 -> [_ _ _ _ _ _ _ _ _ _ _ _ _ _ _]
          tunnel: w302 -> [_ w322 _ w375 w386 w396 _ w420 w457 w470 w484 w506 _ _ _]
          tunnel: w301 -> [_ w320 _ w374 _ w395 w409 w419 _ _ _ _ _ _ _]
          tunnel: w300 -> [_ w309 _ _ _ _ _ _ _ _ _ _ _ _ _]
          frame Default {
          }
          frame "Color Map" {
            w315 = refnum<vi> refnum  # ImageControl
            w311 = u32 5 items=["Grayscale", "Binary", "Gradient", "Rainbow", "Temperature", "User Defined", "Binary 16 Bit", "Gradient 16 Bit", "Rainbow 16 Bit", "Temperature 16 Bit", "User Defined 16 Bit"] ("Palette:Palette Type")
            n168 = for {
              tunnel: w322 -> [w338] mode=indexing
              tunnel: [w339] -> w319
              tunnel: w321 -> [w337]
              i -> [w339]
              stop <- w336 stop-if-true
              n169 = Equal?(x=w337, y=w338) -> (x = y?=w336:bool)
            }
            n170 = Index Array(array=w320, index=w319) -> (element=w318:refnum<vi>)
            n171 = property class="Clust (strict)"(reference=w318) -> ("Controls[]"=w317:refnum<vi>[])  [unwired: 1 in, 2 out]
            n172 = property class="ImageControl"(reference=w321, "Palette Type"=w311) -> (reference out=w323:refnum<vi>)  [unwired: 1 in, 1 out]
            n173 = Index Array(array=w317, index=0) -> (element=w314:refnum<vi>)
            n174 = To More Specific Class(target class=w315, reference=w314) -> (specific class reference=w313:refnum<vi>)  [unwired: 1 in, 1 out]
            n175 = case shown="\"Glow\"" w309 {
              tunnel: [cluster{u8, u8, u8}[] [{0, 0, 0}, {1, 1, 1}, {2, 2, 2}, {3, 3, 3}, {4, 4, 4}, {5, 5, 5}, {6, 6, 6}, {7, 7, 7}, {8, 8, 8}, {9, 9, 9}, {10, 10, 10}, {11, 11, 11}, {12, 12, 12}, {13, 13, 13}, {14, 14, 14}, {15, 15, 15}, {16, 16, 16}, {17, 17, 17}, {18, 18, 18}, {19, 19, 19}, {20, 20, 20}, {21, 21, 21}, {22, 22, 22}, {23, 23, 23}, {24, 24, 24}, {25, 25, 25}, {26, 26, 26}, {27, 27, 27}, {28, 28, 28}, {29, 29, 29}, {30, 30, 30}, {31, 31, 31}, {32, 32, 32}, {33, 33, 33}, {34, 34, 34}, {35, 35, 35}, {36, 36, 36}, {37, 37, 37}, {38, 38, 38}, {39, 39, 39}, {40, 40, 40}, {41, 41, 41}, {42, 42, 42}, {43, 43, 43}, {44, 44, 44}, {45, 45, 45}, {46, 46, 46}, {47, 47, 47}, {48, 48, 48}, {49, 49, 49}, {50, 50, 50}, {51, 51, 51}, {52, 52, 52}, {53, 53, 53}, {54, 54, 54}, {55, 55, 55}, {56, 56, 56}, {57, 57, 57}, {58, 58, 58}, {59, 59, 59}, {60, 60, 60}, {61, 61, 61}, {62, 62, 62}, {63, 63, 63}, {64, 64, 64}, {65, 65, 65}, {66, 66, 66}, {67, 67, 67}, {68, 68, 68}, {69, 69, 69}, {70, 70, 70}, {71, 71, 71}, {72, 72, 72}, {73, 73, 73}, {74, 74, 74}, {75, 75, 75}, {76, 76, 76}, {77, 77, 77}, {78, 78, 78}, {79, 79, 79}, {80, 80, 80}, {81, 81, 81}, {82, 82, 82}, {83, 83, 83}, {84, 84, 84}, {85, 85, 85}, {86, 86, 86}, {87, 87, 87}, {88, 88, 88}, {89, 89, 89}, {90, 90, 90}, {91, 91, 91}, {92, 92, 92}, {93, 93, 93}, {94, 94, 94}, {95, 95, 95}, {96, 96, 96}, {97, 97, 97}, {98, 98, 98}, {99, 99, 99}, {100, 100, 100}, {101, 101, 101}, {102, 102, 102}, {103, 103, 103}, {104, 104, 104}, {105, 105, 105}, {106, 106, 106}, {107, 107, 107}, {108, 108, 108}, {109, 109, 109}, {110, 110, 110}, {111, 111, 111}, {112, 112, 112}, {113, 113, 113}, {114, 114, 114}, {115, 115, 115}, {116, 116, 116}, {117, 117, 117}, {118, 118, 118}, {119, 119, 119}, {120, 120, 120}, {121, 121, 121}, {122, 122, 122}, {123, 123, 123}, {124, 124, 124}, {125, 125, 125}, {126, 126, 126}, {127, 127, 127}, {128, 128, 128}, {129, 129, 129}, {130, 130, 130}, {131, 131, 131}, {132, 132, 132}, {133, 133, 133}, {134, 134, 134}, {135, 135, 135}, {136, 136, 136}, {137, 137, 137}, {138, 138, 138}, {139, 139, 139}, {140, 140, 140}, {141, 141, 141}, {142, 142, 142}, {143, 143, 143}, {144, 144, 144}, {145, 145, 145}, {146, 146, 146}, {147, 147, 147}, {148, 148, 148}, {149, 149, 149}, {150, 150, 150}, {151, 151, 151}, {152, 152, 152}, {153, 153, 153}, {154, 154, 154}, {155, 155, 155}, {156, 156, 156}, {157, 157, 157}, {158, 158, 158}, {159, 159, 159}, {160, 160, 160}, {161, 161, 161}, {162, 162, 162}, {163, 163, 163}, {164, 164, 164}, {165, 165, 165}, {166, 166, 166}, {167, 167, 167}, {168, 168, 168}, {169, 169, 169}, {170, 170, 170}, {171, 171, 171}, {172, 172, 172}, {173, 173, 173}, {174, 174, 174}, {175, 175, 175}, {176, 176, 176}, {177, 177, 177}, {178, 178, 178}, {179, 179, 179}, {180, 180, 180}, {181, 181, 181}, {182, 182, 182}, {183, 183, 183}, {184, 184, 184}, {185, 185, 185}, {186, 186, 186}, {187, 187, 187}, {188, 188, 188}, {189, 189, 189}, {190, 190, 190}, {191, 191, 191}, {192, 192, 192}, {193, 193, 193}, {194, 194, 194}, {195, 195, 195}, {196, 196, 196}, {197, 197, 197}, {198, 198, 198}, {199, 199, 199}, {200, 200, 200}, {201, 201, 201}, {202, 202, 202}, {203, 203, 203}, {204, 204, 204}, {205, 205, 205}, {206, 206, 206}, {207, 207, 207}, {208, 208, 208}, {209, 209, 209}, {210, 210, 210}, {211, 211, 211}, {212, 212, 212}, {213, 213, 213}, {214, 214, 214}, {215, 215, 215}, {216, 216, 216}, {217, 217, 217}, {218, 218, 218}, {219, 219, 219}, {220, 220, 220}, {221, 221, 221}, {222, 222, 222}, {223, 223, 223}, {224, 224, 224}, {225, 225, 225}, {226, 226, 226}, {227, 227, 227}, {228, 228, 228}, {229, 229, 229}, {230, 230, 230}, {231, 231, 231}, {232, 232, 232}, {233, 233, 233}, {234, 234, 234}, {235, 235, 235}, {236, 236, 236}, {237, 237, 237}, {238, 238, 238}, {239, 239, 239}, {240, 240, 240}, {241, 241, 241}, {242, 242, 242}, {243, 243, 243}, {244, 244, 244}, {245, 245, 245}, {246, 246, 246}, {247, 247, 247}, {248, 248, 248}, {249, 249, 249}, {250, 250, 250}, {251, 251, 251}, {252, 252, 252}, {253, 253, 253}, {254, 254, 254}, {255, 255, 255}] ("Array") cluster{u8, u8, u8}[] [{0, 0, 0}, {1, 0, 0}, {2, 0, 0}, {3, 0, 0}, {4, 0, 0}, {5, 0, 0}, {6, 0, 0}, {7, 0, 0}, {8, 0, 0}, {9, 0, 0}, {10, 0, 0}, {11, 0, 0}, {12, 0, 0}, {13, 0, 0}, {14, 0, 0}, {15, 0, 0}, {16, 0, 0}, {17, 0, 0}, {18, 0, 0}, {19, 0, 0}, {20, 0, 0}, {21, 0, 0}, {22, 0, 0}, {23, 0, 0}, {24, 0, 0}, {25, 0, 0}, {26, 0, 0}, {27, 0, 0}, {28, 0, 0}, {29, 0, 0}, {30, 0, 0}, {31, 0, 0}, {32, 0, 0}, {33, 0, 0}, {34, 0, 0}, {35, 0, 0}, {36, 0, 0}, {37, 0, 0}, {38, 0, 0}, {39, 0, 0}, {40, 0, 0}, {41, 0, 0}, {42, 0, 0}, {43, 0, 0}, {44, 0, 0}, {45, 0, 0}, {46, 0, 0}, {47, 0, 0}, {48, 0, 0}, {49, 0, 0}, {50, 0, 0}, {51, 0, 0}, {52, 0, 0}, {53, 0, 0}, {54, 0, 0}, {55, 0, 0}, {56, 0, 0}, {57, 0, 0}, {58, 0, 0}, {59, 0, 0}, {60, 0, 0}, {61, 0, 0}, {62, 0, 0}, {63, 0, 0}, {64, 0, 0}, {65, 0, 0}, {66, 0, 0}, {67, 0, 0}, {68, 0, 0}, {69, 0, 0}, {70, 0, 0}, {71, 0, 0}, {72, 0, 0}, {73, 0, 0}, {74, 0, 0}, {75, 0, 0}, {76, 0, 0}, {77, 0, 0}, {78, 0, 0}, {79, 0, 0}, {80, 0, 0}, {81, 0, 0}, {82, 0, 0}, {83, 0, 0}, {84, 0, 0}, {85, 0, 0}, {86, 0, 0}, {87, 0, 0}, {88, 0, 0}, {89, 0, 0}, {90, 0, 0}, {91, 0, 0}, {92, 0, 0}, {93, 0, 0}, {94, 0, 0}, {95, 0, 0}, {96, 0, 0}, {97, 0, 0}, {98, 0, 0}, {99, 0, 0}, {100, 0, 0}, {101, 0, 0}, {102, 0, 0}, {103, 0, 0}, {104, 0, 0}, {105, 0, 0}, {106, 0, 0}, {107, 0, 0}, {108, 0, 0}, {109, 0, 0}, {110, 0, 0}, {111, 0, 0}, {112, 0, 0}, {113, 0, 0}, {114, 0, 0}, {115, 0, 0}, {116, 0, 0}, {117, 0, 0}, {118, 0, 0}, {119, 0, 0}, {120, 0, 0}, {121, 0, 0}, {122, 0, 0}, {123, 0, 0}, {124, 0, 0}, {125, 0, 0}, {126, 0, 0}, {127, 0, 0}, {128, 0, 0}, {129, 0, 0}, {130, 0, 0}, {131, 0, 0}, {132, 0, 0}, {133, 0, 0}, {134, 0, 0}, {135, 0, 0}, {136, 0, 0}, {137, 0, 0}, {138, 0, 0}, {139, 0, 0}, {140, 0, 0}, {141, 0, 0}, {142, 0, 0}, {143, 0, 0}, {144, 0, 0}, {145, 0, 0}, {146, 0, 0}, {147, 0, 0}, {148, 0, 0}, {149, 0, 0}, {150, 0, 0}, {151, 0, 0}, {152, 0, 0}, {153, 0, 0}, {154, 0, 0}, {155, 0, 0}, {156, 0, 0}, {157, 0, 0}, {158, 0, 0}, {159, 0, 0}, {160, 0, 0}, {161, 0, 0}, {162, 0, 0}, {163, 0, 0}, {164, 0, 0}, {165, 0, 0}, {166, 0, 0}, {167, 0, 0}, {168, 0, 0}, {169, 0, 0}, {170, 0, 0}, {171, 0, 0}, {172, 0, 0}, {173, 0, 0}, {174, 0, 0}, {175, 0, 0}, {176, 0, 0}, {177, 0, 0}, {178, 0, 0}, {179, 0, 0}, {180, 0, 0}, {181, 0, 0}, {182, 0, 0}, {183, 0, 0}, {184, 0, 0}, {185, 0, 0}, {186, 0, 0}, {187, 0, 0}, {188, 0, 0}, {189, 0, 0}, {190, 0, 0}, {191, 0, 0}, {192, 0, 0}, {193, 0, 0}, {194, 0, 0}, {195, 0, 0}, {196, 0, 0}, {197, 0, 0}, {198, 0, 0}, {199, 0, 0}, {200, 0, 0}, {201, 0, 0}, {202, 0, 0}, {203, 0, 0}, {204, 0, 0}, {205, 0, 0}, {206, 0, 0}, {207, 0, 0}, {208, 0, 0}, {209, 0, 0}, {210, 0, 0}, {211, 0, 0}, {212, 0, 0}, {213, 0, 0}, {214, 0, 0}, {215, 0, 0}, {216, 0, 0}, {217, 0, 0}, {218, 0, 0}, {219, 0, 0}, {220, 0, 0}, {221, 0, 0}, {222, 0, 0}, {223, 0, 0}, {224, 0, 0}, {225, 0, 0}, {226, 0, 0}, {227, 0, 0}, {228, 0, 0}, {229, 0, 0}, {230, 0, 0}, {231, 0, 0}, {232, 0, 0}, {233, 0, 0}, {234, 0, 0}, {235, 0, 0}, {236, 0, 0}, {237, 0, 0}, {238, 0, 0}, {239, 0, 0}, {240, 0, 0}, {241, 0, 0}, {242, 0, 0}, {243, 0, 0}, {244, 0, 0}, {245, 0, 0}, {246, 0, 0}, {247, 0, 0}, {248, 0, 0}, {249, 0, 0}, {250, 0, 0}, {251, 0, 0}, {252, 0, 0}, {253, 0, 0}, {254, 0, 0}, {255, 0, 0}] ("Array") cluster{u8, u8, u8}[] [{0, 0, 0}, {0, 1, 0}, {0, 2, 0}, {0, 3, 0}, {0, 4, 0}, {0, 5, 0}, {0, 6, 0}, {0, 7, 0}, {0, 8, 0}, {0, 9, 0}, {0, 10, 0}, {0, 11, 0}, {0, 12, 0}, {0, 13, 0}, {0, 14, 0}, {0, 15, 0}, {0, 16, 0}, {0, 17, 0}, {0, 18, 0}, {0, 19, 0}, {0, 20, 0}, {0, 21, 0}, {0, 22, 0}, {0, 23, 0}, {0, 24, 0}, {0, 25, 0}, {0, 26, 0}, {0, 27, 0}, {0, 28, 0}, {0, 29, 0}, {0, 30, 0}, {0, 31, 0}, {0, 32, 0}, {0, 33, 0}, {0, 34, 0}, {0, 35, 0}, {0, 36, 0}, {0, 37, 0}, {0, 38, 0}, {0, 39, 0}, {0, 40, 0}, {0, 41, 0}, {0, 42, 0}, {0, 43, 0}, {0, 44, 0}, {0, 45, 0}, {0, 46, 0}, {0, 47, 0}, {0, 48, 0}, {0, 49, 0}, {0, 50, 0}, {0, 51, 0}, {0, 52, 0}, {0, 53, 0}, {0, 54, 0}, {0, 55, 0}, {0, 56, 0}, {0, 57, 0}, {0, 58, 0}, {0, 59, 0}, {0, 60, 0}, {0, 61, 0}, {0, 62, 0}, {0, 63, 0}, {0, 64, 0}, {0, 65, 0}, {0, 66, 0}, {0, 67, 0}, {0, 68, 0}, {0, 69, 0}, {0, 70, 0}, {0, 71, 0}, {0, 72, 0}, {0, 73, 0}, {0, 74, 0}, {0, 75, 0}, {0, 76, 0}, {0, 77, 0}, {0, 78, 0}, {0, 79, 0}, {0, 80, 0}, {0, 81, 0}, {0, 82, 0}, {0, 83, 0}, {0, 84, 0}, {0, 85, 0}, {0, 86, 0}, {0, 87, 0}, {0, 88, 0}, {0, 89, 0}, {0, 90, 0}, {0, 91, 0}, {0, 92, 0}, {0, 93, 0}, {0, 94, 0}, {0, 95, 0}, {0, 96, 0}, {0, 97, 0}, {0, 98, 0}, {0, 99, 0}, {0, 100, 0}, {0, 101, 0}, {0, 102, 0}, {0, 103, 0}, {0, 104, 0}, {0, 105, 0}, {0, 106, 0}, {0, 107, 0}, {0, 108, 0}, {0, 109, 0}, {0, 110, 0}, {0, 111, 0}, {0, 112, 0}, {0, 113, 0}, {0, 114, 0}, {0, 115, 0}, {0, 116, 0}, {0, 117, 0}, {0, 118, 0}, {0, 119, 0}, {0, 120, 0}, {0, 121, 0}, {0, 122, 0}, {0, 123, 0}, {0, 124, 0}, {0, 125, 0}, {0, 126, 0}, {0, 127, 0}, {0, 128, 0}, {0, 129, 0}, {0, 130, 0}, {0, 131, 0}, {0, 132, 0}, {0, 133, 0}, {0, 134, 0}, {0, 135, 0}, {0, 136, 0}, {0, 137, 0}, {0, 138, 0}, {0, 139, 0}, {0, 140, 0}, {0, 141, 0}, {0, 142, 0}, {0, 143, 0}, {0, 144, 0}, {0, 145, 0}, {0, 146, 0}, {0, 147, 0}, {0, 148, 0}, {0, 149, 0}, {0, 150, 0}, {0, 151, 0}, {0, 152, 0}, {0, 153, 0}, {0, 154, 0}, {0, 155, 0}, {0, 156, 0}, {0, 157, 0}, {0, 158, 0}, {0, 159, 0}, {0, 160, 0}, {0, 161, 0}, {0, 162, 0}, {0, 163, 0}, {0, 164, 0}, {0, 165, 0}, {0, 166, 0}, {0, 167, 0}, {0, 168, 0}, {0, 169, 0}, {0, 170, 0}, {0, 171, 0}, {0, 172, 0}, {0, 173, 0}, {0, 174, 0}, {0, 175, 0}, {0, 176, 0}, {0, 177, 0}, {0, 178, 0}, {0, 179, 0}, {0, 180, 0}, {0, 181, 0}, {0, 182, 0}, {0, 183, 0}, {0, 184, 0}, {0, 185, 0}, {0, 186, 0}, {0, 187, 0}, {0, 188, 0}, {0, 189, 0}, {0, 190, 0}, {0, 191, 0}, {0, 192, 0}, {0, 193, 0}, {0, 194, 0}, {0, 195, 0}, {0, 196, 0}, {0, 197, 0}, {0, 198, 0}, {0, 199, 0}, {0, 200, 0}, {0, 201, 0}, {0, 202, 0}, {0, 203, 0}, {0, 204, 0}, {0, 205, 0}, {0, 206, 0}, {0, 207, 0}, {0, 208, 0}, {0, 209, 0}, {0, 210, 0}, {0, 211, 0}, {0, 212, 0}, {0, 213, 0}, {0, 214, 0}, {0, 215, 0}, {0, 216, 0}, {0, 217, 0}, {0, 218, 0}, {0, 219, 0}, {0, 220, 0}, {0, 221, 0}, {0, 222, 0}, {0, 223, 0}, {0, 224, 0}, {0, 225, 0}, {0, 226, 0}, {0, 227, 0}, {0, 228, 0}, {0, 229, 0}, {0, 230, 0}, {0, 231, 0}, {0, 232, 0}, {0, 233, 0}, {0, 234, 0}, {0, 235, 0}, {0, 236, 0}, {0, 237, 0}, {0, 238, 0}, {0, 239, 0}, {0, 240, 0}, {0, 241, 0}, {0, 242, 0}, {0, 243, 0}, {0, 244, 0}, {0, 245, 0}, {0, 246, 0}, {0, 247, 0}, {0, 248, 0}, {0, 249, 0}, {0, 250, 0}, {0, 251, 0}, {0, 252, 0}, {0, 253, 0}, {0, 254, 0}, {0, 255, 0}] ("Array") cluster{u8, u8, u8}[] [{0, 0, 0}, {0, 0, 1}, {0, 0, 2}, {0, 0, 3}, {0, 0, 4}, {0, 0, 5}, {0, 0, 6}, {0, 0, 7}, {0, 0, 8}, {0, 0, 9}, {0, 0, 10}, {0, 0, 11}, {0, 0, 12}, {0, 0, 13}, {0, 0, 14}, {0, 0, 15}, {0, 0, 16}, {0, 0, 17}, {0, 0, 18}, {0, 0, 19}, {0, 0, 20}, {0, 0, 21}, {0, 0, 22}, {0, 0, 23}, {0, 0, 24}, {0, 0, 25}, {0, 0, 26}, {0, 0, 27}, {0, 0, 28}, {0, 0, 29}, {0, 0, 30}, {0, 0, 31}, {0, 0, 32}, {0, 0, 33}, {0, 0, 34}, {0, 0, 35}, {0, 0, 36}, {0, 0, 37}, {0, 0, 38}, {0, 0, 39}, {0, 0, 40}, {0, 0, 41}, {0, 0, 42}, {0, 0, 43}, {0, 0, 44}, {0, 0, 45}, {0, 0, 46}, {0, 0, 47}, {0, 0, 48}, {0, 0, 49}, {0, 0, 50}, {0, 0, 51}, {0, 0, 52}, {0, 0, 53}, {0, 0, 54}, {0, 0, 55}, {0, 0, 56}, {0, 0, 57}, {0, 0, 58}, {0, 0, 59}, {0, 0, 60}, {0, 0, 61}, {0, 0, 62}, {0, 0, 63}, {0, 0, 64}, {0, 0, 65}, {0, 0, 66}, {0, 0, 67}, {0, 0, 68}, {0, 0, 69}, {0, 0, 70}, {0, 0, 71}, {0, 0, 72}, {0, 0, 73}, {0, 0, 74}, {0, 0, 75}, {0, 0, 76}, {0, 0, 77}, {0, 0, 78}, {0, 0, 79}, {0, 0, 80}, {0, 0, 81}, {0, 0, 82}, {0, 0, 83}, {0, 0, 84}, {0, 0, 85}, {0, 0, 86}, {0, 0, 87}, {0, 0, 88}, {0, 0, 89}, {0, 0, 90}, {0, 0, 91}, {0, 0, 92}, {0, 0, 93}, {0, 0, 94}, {0, 0, 95}, {0, 0, 96}, {0, 0, 97}, {0, 0, 98}, {0, 0, 99}, {0, 0, 100}, {0, 0, 101}, {0, 0, 102}, {0, 0, 103}, {0, 0, 104}, {0, 0, 105}, {0, 0, 106}, {0, 0, 107}, {0, 0, 108}, {0, 0, 109}, {0, 0, 110}, {0, 0, 111}, {0, 0, 112}, {0, 0, 113}, {0, 0, 114}, {0, 0, 115}, {0, 0, 116}, {0, 0, 117}, {0, 0, 118}, {0, 0, 119}, {0, 0, 120}, {0, 0, 121}, {0, 0, 122}, {0, 0, 123}, {0, 0, 124}, {0, 0, 125}, {0, 0, 126}, {0, 0, 127}, {0, 0, 128}, {0, 0, 129}, {0, 0, 130}, {0, 0, 131}, {0, 0, 132}, {0, 0, 133}, {0, 0, 134}, {0, 0, 135}, {0, 0, 136}, {0, 0, 137}, {0, 0, 138}, {0, 0, 139}, {0, 0, 140}, {0, 0, 141}, {0, 0, 142}, {0, 0, 143}, {0, 0, 144}, {0, 0, 145}, {0, 0, 146}, {0, 0, 147}, {0, 0, 148}, {0, 0, 149}, {0, 0, 150}, {0, 0, 151}, {0, 0, 152}, {0, 0, 153}, {0, 0, 154}, {0, 0, 155}, {0, 0, 156}, {0, 0, 157}, {0, 0, 158}, {0, 0, 159}, {0, 0, 160}, {0, 0, 161}, {0, 0, 162}, {0, 0, 163}, {0, 0, 164}, {0, 0, 165}, {0, 0, 166}, {0, 0, 167}, {0, 0, 168}, {0, 0, 169}, {0, 0, 170}, {0, 0, 171}, {0, 0, 172}, {0, 0, 173}, {0, 0, 174}, {0, 0, 175}, {0, 0, 176}, {0, 0, 177}, {0, 0, 178}, {0, 0, 179}, {0, 0, 180}, {0, 0, 181}, {0, 0, 182}, {0, 0, 183}, {0, 0, 184}, {0, 0, 185}, {0, 0, 186}, {0, 0, 187}, {0, 0, 188}, {0, 0, 189}, {0, 0, 190}, {0, 0, 191}, {0, 0, 192}, {0, 0, 193}, {0, 0, 194}, {0, 0, 195}, {0, 0, 196}, {0, 0, 197}, {0, 0, 198}, {0, 0, 199}, {0, 0, 200}, {0, 0, 201}, {0, 0, 202}, {0, 0, 203}, {0, 0, 204}, {0, 0, 205}, {0, 0, 206}, {0, 0, 207}, {0, 0, 208}, {0, 0, 209}, {0, 0, 210}, {0, 0, 211}, {0, 0, 212}, {0, 0, 213}, {0, 0, 214}, {0, 0, 215}, {0, 0, 216}, {0, 0, 217}, {0, 0, 218}, {0, 0, 219}, {0, 0, 220}, {0, 0, 221}, {0, 0, 222}, {0, 0, 223}, {0, 0, 224}, {0, 0, 225}, {0, 0, 226}, {0, 0, 227}, {0, 0, 228}, {0, 0, 229}, {0, 0, 230}, {0, 0, 231}, {0, 0, 232}, {0, 0, 233}, {0, 0, 234}, {0, 0, 235}, {0, 0, 236}, {0, 0, 237}, {0, 0, 238}, {0, 0, 239}, {0, 0, 240}, {0, 0, 241}, {0, 0, 242}, {0, 0, 243}, {0, 0, 244}, {0, 0, 245}, {0, 0, 246}, {0, 0, 247}, {0, 0, 248}, {0, 0, 249}, {0, 0, 250}, {0, 0, 251}, {0, 0, 252}, {0, 0, 253}, {0, 0, 254}, {0, 0, 255}] ("Array") cluster{u8, u8, u8}[] [{0, 0, 0}, {0, 1, 1}, {0, 2, 2}, {0, 3, 3}, {0, 4, 4}, {0, 5, 5}, {0, 6, 6}, {0, 7, 7}, {0, 8, 8}, {0, 9, 9}, {0, 10, 10}, {0, 11, 11}, {0, 12, 12}, {0, 13, 13}, {0, 14, 14}, {0, 15, 15}, {0, 16, 16}, {0, 17, 17}, {0, 18, 18}, {0, 19, 19}, {0, 20, 20}, {0, 21, 21}, {0, 22, 22}, {0, 23, 23}, {0, 24, 24}, {0, 25, 25}, {0, 26, 26}, {0, 27, 27}, {0, 28, 28}, {0, 29, 29}, {0, 30, 30}, {0, 31, 31}, {0, 32, 32}, {0, 33, 33}, {0, 34, 34}, {0, 35, 35}, {0, 36, 36}, {0, 37, 37}, {0, 38, 38}, {0, 39, 39}, {0, 40, 40}, {0, 41, 41}, {0, 42, 42}, {0, 43, 43}, {0, 44, 44}, {0, 45, 45}, {0, 46, 46}, {0, 47, 47}, {0, 48, 48}, {0, 49, 49}, {0, 50, 50}, {0, 51, 51}, {0, 52, 52}, {0, 53, 53}, {0, 54, 54}, {0, 55, 55}, {0, 56, 56}, {0, 57, 57}, {0, 58, 58}, {0, 59, 59}, {0, 60, 60}, {0, 61, 61}, {0, 62, 62}, {0, 63, 63}, {0, 64, 64}, {0, 65, 65}, {0, 66, 66}, {0, 67, 67}, {0, 68, 68}, {0, 69, 69}, {0, 70, 70}, {0, 71, 71}, {0, 72, 72}, {0, 73, 73}, {0, 74, 74}, {0, 75, 75}, {0, 76, 76}, {0, 77, 77}, {0, 78, 78}, {0, 79, 79}, {0, 80, 80}, {0, 81, 81}, {0, 82, 82}, {0, 83, 83}, {0, 84, 84}, {0, 85, 85}, {0, 86, 86}, {0, 87, 87}, {0, 88, 88}, {0, 89, 89}, {0, 90, 90}, {0, 91, 91}, {0, 92, 92}, {0, 93, 93}, {0, 94, 94}, {0, 95, 95}, {0, 96, 96}, {0, 97, 97}, {0, 98, 98}, {0, 99, 99}, {0, 100, 100}, {0, 101, 101}, {0, 102, 102}, {0, 103, 103}, {0, 104, 104}, {0, 105, 105}, {0, 106, 106}, {0, 107, 107}, {0, 108, 108}, {0, 109, 109}, {0, 110, 110}, {0, 111, 111}, {0, 112, 112}, {0, 113, 113}, {0, 114, 114}, {0, 115, 115}, {0, 116, 116}, {0, 117, 117}, {0, 118, 118}, {0, 119, 119}, {0, 120, 120}, {0, 121, 121}, {0, 122, 122}, {0, 123, 123}, {0, 124, 124}, {0, 125, 125}, {0, 126, 126}, {0, 127, 127}, {0, 128, 128}, {0, 129, 129}, {0, 130, 130}, {0, 131, 131}, {0, 132, 132}, {0, 133, 133}, {0, 134, 134}, {0, 135, 135}, {0, 136, 136}, {0, 137, 137}, {0, 138, 138}, {0, 139, 139}, {0, 140, 140}, {0, 141, 141}, {0, 142, 142}, {0, 143, 143}, {0, 144, 144}, {0, 145, 145}, {0, 146, 146}, {0, 147, 147}, {0, 148, 148}, {0, 149, 149}, {0, 150, 150}, {0, 151, 151}, {0, 152, 152}, {0, 153, 153}, {0, 154, 154}, {0, 155, 155}, {0, 156, 156}, {0, 157, 157}, {0, 158, 158}, {0, 159, 159}, {0, 160, 160}, {0, 161, 161}, {0, 162, 162}, {0, 163, 163}, {0, 164, 164}, {0, 165, 165}, {0, 166, 166}, {0, 167, 167}, {0, 168, 168}, {0, 169, 169}, {0, 170, 170}, {0, 171, 171}, {0, 172, 172}, {0, 173, 173}, {0, 174, 174}, {0, 175, 175}, {0, 176, 176}, {0, 177, 177}, {0, 178, 178}, {0, 179, 179}, {0, 180, 180}, {0, 181, 181}, {0, 182, 182}, {0, 183, 183}, {0, 184, 184}, {0, 185, 185}, {0, 186, 186}, {0, 187, 187}, {0, 188, 188}, {0, 189, 189}, {0, 190, 190}, {0, 191, 191}, {0, 192, 192}, {0, 193, 193}, {0, 194, 194}, {0, 195, 195}, {0, 196, 196}, {0, 197, 197}, {0, 198, 198}, {0, 199, 199}, {0, 200, 200}, {0, 201, 201}, {0, 202, 202}, {0, 203, 203}, {0, 204, 204}, {0, 205, 205}, {0, 206, 206}, {0, 207, 207}, {0, 208, 208}, {0, 209, 209}, {0, 210, 210}, {0, 211, 211}, {0, 212, 212}, {0, 213, 213}, {0, 214, 214}, {0, 215, 215}, {0, 216, 216}, {0, 217, 217}, {0, 218, 218}, {0, 219, 219}, {0, 220, 220}, {0, 221, 221}, {0, 222, 222}, {0, 223, 223}, {0, 224, 224}, {0, 225, 225}, {0, 226, 226}, {0, 227, 227}, {0, 228, 228}, {0, 229, 229}, {0, 230, 230}, {0, 231, 231}, {0, 232, 232}, {0, 233, 233}, {0, 234, 234}, {0, 235, 235}, {0, 236, 236}, {0, 237, 237}, {0, 238, 238}, {0, 239, 239}, {0, 240, 240}, {0, 241, 241}, {0, 242, 242}, {0, 243, 243}, {0, 244, 244}, {0, 245, 245}, {0, 246, 246}, {0, 247, 247}, {0, 248, 248}, {0, 249, 249}, {0, 250, 250}, {0, 251, 251}, {0, 252, 252}, {0, 253, 253}, {0, 254, 254}, {0, 255, 255}] ("Array") cluster{u8, u8, u8}[] [{0, 0, 0}, {1, 0, 1}, {2, 0, 2}, {3, 0, 3}, {4, 0, 4}, {5, 0, 5}, {6, 0, 6}, {7, 0, 7}, {8, 0, 8}, {9, 0, 9}, {10, 0, 10}, {11, 0, 11}, {12, 0, 12}, {13, 0, 13}, {14, 0, 14}, {15, 0, 15}, {16, 0, 16}, {17, 0, 17}, {18, 0, 18}, {19, 0, 19}, {20, 0, 20}, {21, 0, 21}, {22, 0, 22}, {23, 0, 23}, {24, 0, 24}, {25, 0, 25}, {26, 0, 26}, {27, 0, 27}, {28, 0, 28}, {29, 0, 29}, {30, 0, 30}, {31, 0, 31}, {32, 0, 32}, {33, 0, 33}, {34, 0, 34}, {35, 0, 35}, {36, 0, 36}, {37, 0, 37}, {38, 0, 38}, {39, 0, 39}, {40, 0, 40}, {41, 0, 41}, {42, 0, 42}, {43, 0, 43}, {44, 0, 44}, {45, 0, 45}, {46, 0, 46}, {47, 0, 47}, {48, 0, 48}, {49, 0, 49}, {50, 0, 50}, {51, 0, 51}, {52, 0, 52}, {53, 0, 53}, {54, 0, 54}, {55, 0, 55}, {56, 0, 56}, {57, 0, 57}, {58, 0, 58}, {59, 0, 59}, {60, 0, 60}, {61, 0, 61}, {62, 0, 62}, {63, 0, 63}, {64, 0, 64}, {65, 0, 65}, {66, 0, 66}, {67, 0, 67}, {68, 0, 68}, {69, 0, 69}, {70, 0, 70}, {71, 0, 71}, {72, 0, 72}, {73, 0, 73}, {74, 0, 74}, {75, 0, 75}, {76, 0, 76}, {77, 0, 77}, {78, 0, 78}, {79, 0, 79}, {80, 0, 80}, {81, 0, 81}, {82, 0, 82}, {83, 0, 83}, {84, 0, 84}, {85, 0, 85}, {86, 0, 86}, {87, 0, 87}, {88, 0, 88}, {89, 0, 89}, {90, 0, 90}, {91, 0, 91}, {92, 0, 92}, {93, 0, 93}, {94, 0, 94}, {95, 0, 95}, {96, 0, 96}, {97, 0, 97}, {98, 0, 98}, {99, 0, 99}, {100, 0, 100}, {101, 0, 101}, {102, 0, 102}, {103, 0, 103}, {104, 0, 104}, {105, 0, 105}, {106, 0, 106}, {107, 0, 107}, {108, 0, 108}, {109, 0, 109}, {110, 0, 110}, {111, 0, 111}, {112, 0, 112}, {113, 0, 113}, {114, 0, 114}, {115, 0, 115}, {116, 0, 116}, {117, 0, 117}, {118, 0, 118}, {119, 0, 119}, {120, 0, 120}, {121, 0, 121}, {122, 0, 122}, {123, 0, 123}, {124, 0, 124}, {125, 0, 125}, {126, 0, 126}, {127, 0, 127}, {128, 0, 128}, {129, 0, 129}, {130, 0, 130}, {131, 0, 131}, {132, 0, 132}, {133, 0, 133}, {134, 0, 134}, {135, 0, 135}, {136, 0, 136}, {137, 0, 137}, {138, 0, 138}, {139, 0, 139}, {140, 0, 140}, {141, 0, 141}, {142, 0, 142}, {143, 0, 143}, {144, 0, 144}, {145, 0, 145}, {146, 0, 146}, {147, 0, 147}, {148, 0, 148}, {149, 0, 149}, {150, 0, 150}, {151, 0, 151}, {152, 0, 152}, {153, 0, 153}, {154, 0, 154}, {155, 0, 155}, {156, 0, 156}, {157, 0, 157}, {158, 0, 158}, {159, 0, 159}, {160, 0, 160}, {161, 0, 161}, {162, 0, 162}, {163, 0, 163}, {164, 0, 164}, {165, 0, 165}, {166, 0, 166}, {167, 0, 167}, {168, 0, 168}, {169, 0, 169}, {170, 0, 170}, {171, 0, 171}, {172, 0, 172}, {173, 0, 173}, {174, 0, 174}, {175, 0, 175}, {176, 0, 176}, {177, 0, 177}, {178, 0, 178}, {179, 0, 179}, {180, 0, 180}, {181, 0, 181}, {182, 0, 182}, {183, 0, 183}, {184, 0, 184}, {185, 0, 185}, {186, 0, 186}, {187, 0, 187}, {188, 0, 188}, {189, 0, 189}, {190, 0, 190}, {191, 0, 191}, {192, 0, 192}, {193, 0, 193}, {194, 0, 194}, {195, 0, 195}, {196, 0, 196}, {197, 0, 197}, {198, 0, 198}, {199, 0, 199}, {200, 0, 200}, {201, 0, 201}, {202, 0, 202}, {203, 0, 203}, {204, 0, 204}, {205, 0, 205}, {206, 0, 206}, {207, 0, 207}, {208, 0, 208}, {209, 0, 209}, {210, 0, 210}, {211, 0, 211}, {212, 0, 212}, {213, 0, 213}, {214, 0, 214}, {215, 0, 215}, {216, 0, 216}, {217, 0, 217}, {218, 0, 218}, {219, 0, 219}, {220, 0, 220}, {221, 0, 221}, {222, 0, 222}, {223, 0, 223}, {224, 0, 224}, {225, 0, 225}, {226, 0, 226}, {227, 0, 227}, {228, 0, 228}, {229, 0, 229}, {230, 0, 230}, {231, 0, 231}, {232, 0, 232}, {233, 0, 233}, {234, 0, 234}, {235, 0, 235}, {236, 0, 236}, {237, 0, 237}, {238, 0, 238}, {239, 0, 239}, {240, 0, 240}, {241, 0, 241}, {242, 0, 242}, {243, 0, 243}, {244, 0, 244}, {245, 0, 245}, {246, 0, 246}, {247, 0, 247}, {248, 0, 248}, {249, 0, 249}, {250, 0, 250}, {251, 0, 251}, {252, 0, 252}, {253, 0, 253}, {254, 0, 254}, {255, 0, 255}] ("Array") cluster{u8, u8, u8}[] [{0, 0, 0}, {1, 1, 0}, {2, 2, 0}, {3, 3, 0}, {4, 4, 0}, {5, 5, 0}, {6, 6, 0}, {7, 7, 0}, {8, 8, 0}, {9, 9, 0}, {10, 10, 0}, {11, 11, 0}, {12, 12, 0}, {13, 13, 0}, {14, 14, 0}, {15, 15, 0}, {16, 16, 0}, {17, 17, 0}, {18, 18, 0}, {19, 19, 0}, {20, 20, 0}, {21, 21, 0}, {22, 22, 0}, {23, 23, 0}, {24, 24, 0}, {25, 25, 0}, {26, 26, 0}, {27, 27, 0}, {28, 28, 0}, {29, 29, 0}, {30, 30, 0}, {31, 31, 0}, {32, 32, 0}, {33, 33, 0}, {34, 34, 0}, {35, 35, 0}, {36, 36, 0}, {37, 37, 0}, {38, 38, 0}, {39, 39, 0}, {40, 40, 0}, {41, 41, 0}, {42, 42, 0}, {43, 43, 0}, {44, 44, 0}, {45, 45, 0}, {46, 46, 0}, {47, 47, 0}, {48, 48, 0}, {49, 49, 0}, {50, 50, 0}, {51, 51, 0}, {52, 52, 0}, {53, 53, 0}, {54, 54, 0}, {55, 55, 0}, {56, 56, 0}, {57, 57, 0}, {58, 58, 0}, {59, 59, 0}, {60, 60, 0}, {61, 61, 0}, {62, 62, 0}, {63, 63, 0}, {64, 64, 0}, {65, 65, 0}, {66, 66, 0}, {67, 67, 0}, {68, 68, 0}, {69, 69, 0}, {70, 70, 0}, {71, 71, 0}, {72, 72, 0}, {73, 73, 0}, {74, 74, 0}, {75, 75, 0}, {76, 76, 0}, {77, 77, 0}, {78, 78, 0}, {79, 79, 0}, {80, 80, 0}, {81, 81, 0}, {82, 82, 0}, {83, 83, 0}, {84, 84, 0}, {85, 85, 0}, {86, 86, 0}, {87, 87, 0}, {88, 88, 0}, {89, 89, 0}, {90, 90, 0}, {91, 91, 0}, {92, 92, 0}, {93, 93, 0}, {94, 94, 0}, {95, 95, 0}, {96, 96, 0}, {97, 97, 0}, {98, 98, 0}, {99, 99, 0}, {100, 100, 0}, {101, 101, 0}, {102, 102, 0}, {103, 103, 0}, {104, 104, 0}, {105, 105, 0}, {106, 106, 0}, {107, 107, 0}, {108, 108, 0}, {109, 109, 0}, {110, 110, 0}, {111, 111, 0}, {112, 112, 0}, {113, 113, 0}, {114, 114, 0}, {115, 115, 0}, {116, 116, 0}, {117, 117, 0}, {118, 118, 0}, {119, 119, 0}, {120, 120, 0}, {121, 121, 0}, {122, 122, 0}, {123, 123, 0}, {124, 124, 0}, {125, 125, 0}, {126, 126, 0}, {127, 127, 0}, {128, 128, 0}, {129, 129, 0}, {130, 130, 0}, {131, 131, 0}, {132, 132, 0}, {133, 133, 0}, {134, 134, 0}, {135, 135, 0}, {136, 136, 0}, {137, 137, 0}, {138, 138, 0}, {139, 139, 0}, {140, 140, 0}, {141, 141, 0}, {142, 142, 0}, {143, 143, 0}, {144, 144, 0}, {145, 145, 0}, {146, 146, 0}, {147, 147, 0}, {148, 148, 0}, {149, 149, 0}, {150, 150, 0}, {151, 151, 0}, {152, 152, 0}, {153, 153, 0}, {154, 154, 0}, {155, 155, 0}, {156, 156, 0}, {157, 157, 0}, {158, 158, 0}, {159, 159, 0}, {160, 160, 0}, {161, 161, 0}, {162, 162, 0}, {163, 163, 0}, {164, 164, 0}, {165, 165, 0}, {166, 166, 0}, {167, 167, 0}, {168, 168, 0}, {169, 169, 0}, {170, 170, 0}, {171, 171, 0}, {172, 172, 0}, {173, 173, 0}, {174, 174, 0}, {175, 175, 0}, {176, 176, 0}, {177, 177, 0}, {178, 178, 0}, {179, 179, 0}, {180, 180, 0}, {181, 181, 0}, {182, 182, 0}, {183, 183, 0}, {184, 184, 0}, {185, 185, 0}, {186, 186, 0}, {187, 187, 0}, {188, 188, 0}, {189, 189, 0}, {190, 190, 0}, {191, 191, 0}, {192, 192, 0}, {193, 193, 0}, {194, 194, 0}, {195, 195, 0}, {196, 196, 0}, {197, 197, 0}, {198, 198, 0}, {199, 199, 0}, {200, 200, 0}, {201, 201, 0}, {202, 202, 0}, {203, 203, 0}, {204, 204, 0}, {205, 205, 0}, {206, 206, 0}, {207, 207, 0}, {208, 208, 0}, {209, 209, 0}, {210, 210, 0}, {211, 211, 0}, {212, 212, 0}, {213, 213, 0}, {214, 214, 0}, {215, 215, 0}, {216, 216, 0}, {217, 217, 0}, {218, 218, 0}, {219, 219, 0}, {220, 220, 0}, {221, 221, 0}, {222, 222, 0}, {223, 223, 0}, {224, 224, 0}, {225, 225, 0}, {226, 226, 0}, {227, 227, 0}, {228, 228, 0}, {229, 229, 0}, {230, 230, 0}, {231, 231, 0}, {232, 232, 0}, {233, 233, 0}, {234, 234, 0}, {235, 235, 0}, {236, 236, 0}, {237, 237, 0}, {238, 238, 0}, {239, 239, 0}, {240, 240, 0}, {241, 241, 0}, {242, 242, 0}, {243, 243, 0}, {244, 244, 0}, {245, 245, 0}, {246, 246, 0}, {247, 247, 0}, {248, 248, 0}, {249, 249, 0}, {250, 250, 0}, {251, 251, 0}, {252, 252, 0}, {253, 253, 0}, {254, 254, 0}, {255, 255, 0}] ("Array") cluster{u8, u8, u8}[] [{0, 0, 0}, {2, 0, 0}, {3, 0, 0}, {4, 0, 0}, {6, 0, 0}, {8, 0, 0}, {9, 0, 0}, {10, 0, 0}, {12, 0, 0}, {14, 0, 0}, {15, 0, 0}, {16, 0, 0}, {18, 0, 0}, {20, 0, 0}, {21, 0, 0}, {22, 0, 0}, {24, 0, 0}, {26, 0, 0}, {27, 0, 0}, {28, 0, 0}, {30, 0, 0}, {32, 0, 0}, {33, 0, 0}, {34, 0, 0}, {36, 0, 0}, {38, 0, 0}, {39, 0, 0}, {40, 0, 0}, {42, 0, 0}, {44, 0, 0}, {45, 0, 0}, {46, 0, 0}, {48, 0, 0}, {50, 0, 0}, {51, 0, 0}, {52, 0, 0}, {54, 0, 0}, {56, 0, 0}, {57, 0, 0}, {58, 0, 0}, {60, 0, 0}, {62, 0, 0}, {63, 0, 0}, {64, 0, 0}, {66, 0, 0}, {68, 0, 0}, {69, 0, 0}, {70, 0, 0}, {72, 0, 0}, {74, 0, 0}, {75, 0, 0}, {76, 0, 0}, {78, 0, 0}, {80, 0, 0}, {81, 0, 0}, {82, 0, 0}, {84, 0, 0}, {86, 0, 0}, {87, 0, 0}, {88, 0, 0}, {90, 0, 0}, {92, 0, 0}, {93, 0, 0}, {94, 0, 0}, {96, 0, 0}, {98, 0, 0}, {99, 0, 0}, {100, 0, 0}, {102, 0, 0}, {104, 0, 0}, {105, 0, 0}, {106, 0, 0}, {108, 0, 0}, {110, 0, 0}, {111, 0, 0}, {112, 0, 0}, {114, 0, 0}, {116, 0, 0}, {117, 0, 0}, {118, 0, 0}, {120, 0, 0}, {122, 0, 0}, {123, 0, 0}, {124, 0, 0}, {126, 0, 0}, {128, 0, 0}, {129, 0, 0}, {130, 0, 0}, {132, 0, 0}, {134, 0, 0}, {135, 0, 0}, {136, 0, 0}, {138, 0, 0}, {140, 0, 0}, {141, 0, 0}, {142, 0, 0}, {144, 0, 0}, {146, 0, 0}, {147, 0, 0}, {148, 0, 0}, {150, 0, 0}, {152, 0, 0}, {153, 0, 0}, {154, 0, 0}, {156, 0, 0}, {158, 0, 0}, {159, 0, 0}, {160, 0, 0}, {162, 0, 0}, {164, 0, 0}, {165, 0, 0}, {166, 0, 0}, {168, 0, 0}, {170, 0, 0}, {171, 0, 0}, {172, 0, 0}, {174, 0, 0}, {176, 0, 0}, {177, 0, 0}, {178, 0, 0}, {180, 0, 0}, {182, 0, 0}, {183, 0, 0}, {184, 0, 0}, {186, 0, 0}, {188, 0, 0}, {189, 0, 0}, {190, 0, 0}, {192, 0, 0}, {194, 0, 0}, {195, 0, 0}, {196, 0, 0}, {198, 0, 0}, {200, 0, 0}, {201, 0, 0}, {202, 0, 0}, {204, 0, 0}, {206, 0, 0}, {207, 0, 0}, {208, 0, 0}, {210, 0, 0}, {212, 0, 0}, {213, 0, 0}, {214, 0, 0}, {216, 0, 0}, {218, 0, 0}, {219, 0, 0}, {220, 0, 0}, {222, 0, 0}, {224, 0, 0}, {225, 0, 0}, {226, 0, 0}, {228, 0, 0}, {230, 0, 0}, {231, 0, 0}, {232, 0, 0}, {234, 0, 0}, {236, 0, 0}, {237, 0, 0}, {238, 0, 0}, {240, 0, 0}, {242, 0, 0}, {243, 0, 0}, {244, 0, 0}, {246, 0, 0}, {248, 0, 0}, {249, 0, 0}, {250, 0, 0}, {252, 0, 0}, {254, 0, 0}, {255, 0, 0}, {255, 3, 3}, {255, 7, 6}, {255, 10, 9}, {255, 14, 12}, {255, 17, 15}, {255, 20, 18}, {255, 24, 21}, {255, 27, 24}, {255, 31, 27}, {255, 34, 30}, {255, 37, 33}, {255, 41, 36}, {255, 44, 39}, {255, 48, 42}, {255, 51, 45}, {255, 54, 48}, {255, 58, 51}, {255, 61, 54}, {255, 65, 57}, {255, 68, 60}, {255, 71, 63}, {255, 75, 66}, {255, 78, 69}, {255, 82, 72}, {255, 85, 75}, {255, 88, 78}, {255, 92, 81}, {255, 95, 84}, {255, 99, 87}, {255, 102, 90}, {255, 105, 93}, {255, 109, 96}, {255, 112, 99}, {255, 116, 102}, {255, 119, 105}, {255, 122, 108}, {255, 126, 111}, {255, 129, 113}, {255, 133, 116}, {255, 136, 119}, {255, 139, 122}, {255, 143, 125}, {255, 146, 128}, {255, 150, 131}, {255, 153, 134}, {255, 156, 137}, {255, 160, 140}, {255, 163, 143}, {255, 167, 146}, {255, 170, 149}, {255, 173, 152}, {255, 177, 155}, {255, 180, 158}, {255, 184, 161}, {255, 187, 164}, {255, 190, 167}, {255, 194, 170}, {255, 197, 173}, {255, 201, 176}, {255, 204, 179}, {255, 207, 182}, {255, 211, 185}, {255, 214, 188}, {255, 218, 191}, {255, 221, 194}, {255, 224, 197}, {255, 228, 200}, {255, 231, 203}, {255, 235, 206}, {255, 238, 209}, {255, 241, 212}, {255, 245, 215}, {255, 248, 218}, {255, 252, 221}, {255, 255, 224}, {255, 255, 227}, {255, 255, 230}, {255, 255, 234}, {255, 255, 237}, {255, 255, 240}, {254, 254, 242}, {253, 253, 244}, {252, 252, 246}, {251, 251, 248}, {250, 250, 250}] ("Array 2") cluster{u8, u8, u8}[] [{0, 0, 0}, {0, 2, 0}, {0, 3, 0}, {0, 4, 0}, {0, 6, 0}, {0, 8, 0}, {0, 9, 0}, {0, 10, 0}, {0, 12, 0}, {0, 14, 0}, {0, 15, 0}, {0, 16, 0}, {0, 18, 0}, {0, 20, 0}, {0, 21, 0}, {0, 22, 0}, {0, 24, 0}, {0, 26, 0}, {0, 27, 0}, {0, 28, 0}, {0, 30, 0}, {0, 32, 0}, {0, 33, 0}, {0, 34, 0}, {0, 36, 0}, {0, 38, 0}, {0, 39, 0}, {0, 40, 0}, {0, 42, 0}, {0, 44, 0}, {0, 45, 0}, {0, 46, 0}, {0, 48, 0}, {0, 50, 0}, {0, 51, 0}, {0, 52, 0}, {0, 54, 0}, {0, 56, 0}, {0, 57, 0}, {0, 58, 0}, {0, 60, 0}, {0, 62, 0}, {0, 63, 0}, {0, 64, 0}, {0, 66, 0}, {0, 68, 0}, {0, 69, 0}, {0, 70, 0}, {0, 72, 0}, {0, 74, 0}, {0, 75, 0}, {0, 76, 0}, {0, 78, 0}, {0, 80, 0}, {0, 81, 0}, {0, 82, 0}, {0, 84, 0}, {0, 86, 0}, {0, 87, 0}, {0, 88, 0}, {0, 90, 0}, {0, 92, 0}, {0, 93, 0}, {0, 94, 0}, {0, 96, 0}, {0, 98, 0}, {0, 99, 0}, {0, 100, 0}, {0, 102, 0}, {0, 104, 0}, {0, 105, 0}, {0, 106, 0}, {0, 108, 0}, {0, 110, 0}, {0, 111, 0}, {0, 112, 0}, {0, 114, 0}, {0, 116, 0}, {0, 117, 0}, {0, 118, 0}, {0, 120, 0}, {0, 122, 0}, {0, 123, 0}, {0, 124, 0}, {0, 126, 0}, {0, 128, 0}, {0, 129, 0}, {0, 130, 0}, {0, 132, 0}, {0, 134, 0}, {0, 135, 0}, {0, 136, 0}, {0, 138, 0}, {0, 140, 0}, {0, 141, 0}, {0, 142, 0}, {0, 144, 0}, {0, 146, 0}, {0, 147, 0}, {0, 148, 0}, {0, 150, 0}, {0, 152, 0}, {0, 153, 0}, {0, 154, 0}, {0, 156, 0}, {0, 158, 0}, {0, 159, 0}, {0, 160, 0}, {0, 162, 0}, {0, 164, 0}, {0, 165, 0}, {0, 166, 0}, {0, 168, 0}, {0, 170, 0}, {0, 171, 0}, {0, 172, 0}, {0, 174, 0}, {0, 176, 0}, {0, 177, 0}, {0, 178, 0}, {0, 180, 0}, {0, 182, 0}, {0, 183, 0}, {0, 184, 0}, {0, 186, 0}, {0, 188, 0}, {0, 189, 0}, {0, 190, 0}, {0, 192, 0}, {0, 194, 0}, {0, 195, 0}, {0, 196, 0}, {0, 198, 0}, {0, 200, 0}, {0, 201, 0}, {0, 202, 0}, {0, 204, 0}, {0, 206, 0}, {0, 207, 0}, {0, 208, 0}, {0, 210, 0}, {0, 212, 0}, {0, 213, 0}, {0, 214, 0}, {0, 216, 0}, {0, 218, 0}, {0, 219, 0}, {0, 220, 0}, {0, 222, 0}, {0, 224, 0}, {0, 225, 0}, {0, 226, 0}, {0, 228, 0}, {0, 230, 0}, {0, 231, 0}, {0, 232, 0}, {0, 234, 0}, {0, 236, 0}, {0, 237, 0}, {0, 238, 0}, {0, 240, 0}, {0, 242, 0}, {0, 243, 0}, {0, 244, 0}, {0, 246, 0}, {0, 248, 0}, {0, 249, 0}, {0, 250, 0}, {0, 252, 0}, {0, 254, 0}, {0, 255, 0}, {3, 255, 3}, {7, 255, 6}, {10, 255, 9}, {14, 255, 12}, {17, 255, 15}, {20, 255, 18}, {24, 255, 21}, {27, 255, 24}, {31, 255, 27}, {34, 255, 30}, {37, 255, 33}, {41, 255, 36}, {44, 255, 39}, {48, 255, 42}, {51, 255, 45}, {54, 255, 48}, {58, 255, 51}, {61, 255, 54}, {65, 255, 57}, {68, 255, 60}, {71, 255, 63}, {75, 255, 66}, {78, 255, 69}, {82, 255, 72}, {85, 255, 75}, {88, 255, 78}, {92, 255, 81}, {95, 255, 84}, {99, 255, 87}, {102, 255, 90}, {105, 255, 93}, {109, 255, 96}, {112, 255, 99}, {116, 255, 102}, {119, 255, 105}, {122, 255, 108}, {126, 255, 111}, {129, 255, 113}, {133, 255, 116}, {136, 255, 119}, {139, 255, 122}, {143, 255, 125}, {146, 255, 128}, {150, 255, 131}, {153, 255, 134}, {156, 255, 137}, {160, 255, 140}, {163, 255, 143}, {167, 255, 146}, {170, 255, 149}, {173, 255, 152}, {177, 255, 155}, {180, 255, 158}, {184, 255, 161}, {187, 255, 164}, {190, 255, 167}, {194, 255, 170}, {197, 255, 173}, {201, 255, 176}, {204, 255, 179}, {207, 255, 182}, {211, 255, 185}, {214, 255, 188}, {218, 255, 191}, {221, 255, 194}, {224, 255, 197}, {228, 255, 200}, {231, 255, 203}, {235, 255, 206}, {238, 255, 209}, {241, 255, 212}, {245, 255, 215}, {248, 255, 218}, {252, 255, 221}, {255, 255, 224}, {255, 255, 227}, {255, 255, 230}, {255, 255, 234}, {255, 255, 237}, {255, 255, 240}, {254, 254, 242}, {253, 253, 244}, {252, 252, 246}, {251, 251, 248}, {250, 250, 250}] ("Array 2") cluster{u8, u8, u8}[] [{0, 0, 0}, {0, 0, 2}, {0, 0, 3}, {0, 0, 4}, {0, 0, 6}, {0, 0, 8}, {0, 0, 9}, {0, 0, 10}, {0, 0, 12}, {0, 0, 14}, {0, 0, 15}, {0, 0, 16}, {0, 0, 18}, {0, 0, 20}, {0, 0, 21}, {0, 0, 22}, {0, 0, 24}, {0, 0, 26}, {0, 0, 27}, {0, 0, 28}, {0, 0, 30}, {0, 0, 32}, {0, 0, 33}, {0, 0, 34}, {0, 0, 36}, {0, 0, 38}, {0, 0, 39}, {0, 0, 40}, {0, 0, 42}, {0, 0, 44}, {0, 0, 45}, {0, 0, 46}, {0, 0, 48}, {0, 0, 50}, {0, 0, 51}, {0, 0, 52}, {0, 0, 54}, {0, 0, 56}, {0, 0, 57}, {0, 0, 58}, {0, 0, 60}, {0, 0, 62}, {0, 0, 63}, {0, 0, 64}, {0, 0, 66}, {0, 0, 68}, {0, 0, 69}, {0, 0, 70}, {0, 0, 72}, {0, 0, 74}, {0, 0, 75}, {0, 0, 76}, {0, 0, 78}, {0, 0, 80}, {0, 0, 81}, {0, 0, 82}, {0, 0, 84}, {0, 0, 86}, {0, 0, 87}, {0, 0, 88}, {0, 0, 90}, {0, 0, 92}, {0, 0, 93}, {0, 0, 94}, {0, 0, 96}, {0, 0, 98}, {0, 0, 99}, {0, 0, 100}, {0, 0, 102}, {0, 0, 104}, {0, 0, 105}, {0, 0, 106}, {0, 0, 108}, {0, 0, 110}, {0, 0, 111}, {0, 0, 112}, {0, 0, 114}, {0, 0, 116}, {0, 0, 117}, {0, 0, 118}, {0, 0, 120}, {0, 0, 122}, {0, 0, 123}, {0, 0, 124}, {0, 0, 126}, {0, 0, 128}, {0, 0, 129}, {0, 0, 130}, {0, 0, 132}, {0, 0, 134}, {0, 0, 135}, {0, 0, 136}, {0, 0, 138}, {0, 0, 140}, {0, 0, 141}, {0, 0, 142}, {0, 0, 144}, {0, 0, 146}, {0, 0, 147}, {0, 0, 148}, {0, 0, 150}, {0, 0, 152}, {0, 0, 153}, {0, 0, 154}, {0, 0, 156}, {0, 0, 158}, {0, 0, 159}, {0, 0, 160}, {0, 0, 162}, {0, 0, 164}, {0, 0, 165}, {0, 0, 166}, {0, 0, 168}, {0, 0, 170}, {0, 0, 171}, {0, 0, 172}, {0, 0, 174}, {0, 0, 176}, {0, 0, 177}, {0, 0, 178}, {0, 0, 180}, {0, 0, 182}, {0, 0, 183}, {0, 0, 184}, {0, 0, 186}, {0, 0, 188}, {0, 0, 189}, {0, 0, 190}, {0, 0, 192}, {0, 0, 194}, {0, 0, 195}, {0, 0, 196}, {0, 0, 198}, {0, 0, 200}, {0, 0, 201}, {0, 0, 202}, {0, 0, 204}, {0, 0, 206}, {0, 0, 207}, {0, 0, 208}, {0, 0, 210}, {0, 0, 212}, {0, 0, 213}, {0, 0, 214}, {0, 0, 216}, {0, 0, 218}, {0, 0, 219}, {0, 0, 220}, {0, 0, 222}, {0, 0, 224}, {0, 0, 225}, {0, 0, 226}, {0, 0, 228}, {0, 0, 230}, {0, 0, 231}, {0, 0, 232}, {0, 0, 234}, {0, 0, 236}, {0, 0, 237}, {0, 0, 238}, {0, 0, 240}, {0, 0, 242}, {0, 0, 243}, {0, 0, 244}, {0, 0, 246}, {0, 0, 248}, {0, 0, 249}, {0, 0, 250}, {0, 0, 252}, {0, 0, 254}, {0, 0, 255}, {3, 3, 255}, {7, 7, 254}, {10, 10, 254}, {14, 14, 253}, {17, 17, 253}, {20, 20, 253}, {24, 24, 252}, {27, 27, 252}, {31, 31, 251}, {34, 34, 251}, {37, 37, 250}, {41, 41, 250}, {44, 44, 250}, {48, 48, 249}, {51, 51, 249}, {54, 54, 248}, {58, 58, 248}, {61, 61, 248}, {65, 65, 247}, {68, 68, 247}, {71, 71, 246}, {75, 75, 246}, {78, 78, 245}, {82, 82, 245}, {85, 85, 245}, {88, 88, 244}, {92, 92, 244}, {95, 95, 243}, {99, 99, 243}, {102, 102, 243}, {105, 105, 242}, {109, 109, 242}, {112, 112, 241}, {116, 116, 241}, {119, 119, 241}, {122, 122, 240}, {126, 126, 240}, {129, 129, 239}, {133, 133, 239}, {136, 136, 238}, {139, 139, 238}, {143, 143, 238}, {146, 146, 237}, {150, 150, 237}, {153, 153, 236}, {156, 156, 236}, {160, 160, 236}, {163, 163, 235}, {167, 167, 235}, {170, 170, 234}, {173, 173, 234}, {177, 177, 234}, {180, 180, 233}, {184, 184, 233}, {187, 187, 232}, {190, 190, 232}, {194, 194, 231}, {197, 197, 231}, {201, 201, 231}, {204, 204, 230}, {207, 207, 230}, {211, 211, 229}, {214, 214, 229}, {218, 218, 229}, {221, 221, 228}, {224, 224, 228}, {228, 228, 227}, {231, 231, 227}, {235, 235, 226}, {238, 238, 226}, {241, 241, 226}, {245, 245, 225}, {248, 248, 225}, {252, 252, 224}, {255, 255, 224}, {255, 255, 227}, {255, 255, 230}, {255, 255, 234}, {255, 255, 237}, {255, 255, 240}, {254, 254, 242}, {253, 253, 244}, {252, 252, 246}, {251, 251, 248}, {250, 250, 250}] ("Array 2") cluster{u8, u8, u8}[] [{0, 0, 0}, {3, 0, 0}, {6, 0, 0}, {9, 0, 0}, {12, 0, 0}, {15, 0, 0}, {18, 0, 0}, {21, 0, 0}, {24, 0, 0}, {27, 0, 0}, {30, 0, 0}, {33, 0, 0}, {36, 0, 0}, {39, 0, 0}, {42, 0, 0}, {45, 0, 0}, {48, 0, 0}, {51, 0, 0}, {54, 0, 0}, {57, 0, 0}, {60, 0, 0}, {63, 0, 0}, {66, 0, 0}, {69, 0, 0}, {72, 0, 0}, {75, 0, 0}, {78, 0, 0}, {81, 0, 0}, {84, 0, 0}, {87, 0, 0}, {90, 0, 0}, {93, 0, 0}, {96, 0, 0}, {99, 0, 0}, {102, 0, 0}, {105, 0, 0}, {108, 0, 0}, {111, 0, 0}, {114, 0, 0}, {117, 0, 0}, {120, 0, 0}, {123, 0, 0}, {126, 0, 0}, {129, 0, 0}, {132, 0, 0}, {135, 0, 0}, {138, 0, 0}, {141, 0, 0}, {144, 0, 0}, {147, 0, 0}, {150, 0, 0}, {153, 0, 0}, {156, 0, 0}, {159, 0, 0}, {162, 0, 0}, {165, 0, 0}, {168, 0, 0}, {171, 0, 0}, {174, 0, 0}, {177, 0, 0}, {180, 0, 0}, {183, 0, 0}, {186, 0, 0}, {189, 0, 0}, {192, 0, 0}, {195, 0, 0}, {198, 0, 0}, {201, 0, 0}, {204, 0, 0}, {207, 0, 0}, {210, 0, 0}, {213, 0, 0}, {216, 0, 0}, {219, 0, 0}, {222, 0, 0}, {225, 0, 0}, {228, 0, 0}, {231, 0, 0}, {234, 0, 0}, {237, 0, 0}, {240, 0, 0}, {243, 0, 0}, {246, 0, 0}, {249, 0, 0}, {252, 0, 0}, {255, 0, 0}, {255, 3, 0}, {255, 6, 0}, {255, 9, 0}, {255, 12, 0}, {255, 15, 0}, {255, 18, 0}, {255, 21, 0}, {255, 24, 0}, {255, 27, 0}, {255, 30, 0}, {255, 33, 0}, {255, 36, 0}, {255, 39, 0}, {255, 42, 0}, {255, 45, 0}, {255, 48, 0}, {255, 51, 0}, {255, 54, 0}, {255, 57, 0}, {255, 60, 0}, {255, 63, 0}, {255, 66, 0}, {255, 69, 0}, {255, 72, 0}, {255, 75, 0}, {255, 78, 0}, {255, 81, 0}, {255, 84, 0}, {255, 87, 0}, {255, 90, 0}, {255, 93, 0}, {255, 96, 0}, {255, 100, 0}, {255, 103, 0}, {255, 106, 0}, {255, 109, 0}, {255, 112, 0}, {255, 115, 0}, {255, 118, 0}, {255, 121, 0}, {255, 124, 0}, {255, 127, 0}, {255, 130, 0}, {255, 132, 0}, {255, 135, 0}, {255, 137, 0}, {255, 140, 0}, {255, 143, 0}, {255, 146, 0}, {255, 149, 0}, {255, 152, 0}, {255, 156, 0}, {255, 159, 0}, {255, 162, 0}, {255, 165, 0}, {255, 168, 0}, {255, 171, 0}, {255, 174, 0}, {255, 177, 0}, {255, 180, 0}, {255, 183, 0}, {255, 186, 0}, {255, 189, 0}, {255, 191, 0}, {255, 194, 0}, {255, 197, 0}, {255, 200, 0}, {255, 203, 0}, {255, 206, 0}, {255, 209, 0}, {255, 212, 0}, {255, 215, 0}, {255, 218, 0}, {255, 221, 0}, {255, 224, 0}, {255, 227, 0}, {255, 230, 0}, {255, 233, 0}, {255, 237, 0}, {255, 240, 0}, {255, 243, 0}, {255, 246, 0}, {255, 249, 0}, {255, 252, 0}, {255, 255, 0}, {255, 255, 3}, {255, 255, 6}, {255, 255, 9}, {255, 255, 12}, {255, 255, 15}, {255, 255, 18}, {255, 255, 21}, {255, 255, 24}, {255, 255, 27}, {255, 255, 30}, {255, 255, 33}, {255, 255, 36}, {255, 255, 39}, {255, 255, 42}, {255, 255, 45}, {255, 255, 48}, {255, 255, 51}, {255, 255, 54}, {255, 255, 57}, {255, 255, 60}, {255, 255, 63}, {255, 255, 66}, {255, 255, 69}, {255, 255, 72}, {255, 255, 75}, {255, 255, 78}, {255, 255, 81}, {255, 255, 84}, {255, 255, 87}, {255, 255, 90}, {255, 255, 93}, {255, 255, 96}, {255, 255, 99}, {255, 255, 102}, {255, 255, 105}, {255, 255, 108}, {255, 255, 111}, {255, 255, 113}, {255, 255, 116}, {255, 255, 119}, {255, 255, 122}, {255, 255, 125}, {255, 255, 128}, {255, 255, 131}, {255, 255, 134}, {255, 255, 137}, {255, 255, 140}, {255, 255, 143}, {255, 255, 146}, {255, 255, 149}, {255, 255, 152}, {255, 255, 155}, {255, 255, 158}, {255, 255, 161}, {255, 255, 164}, {255, 255, 167}, {255, 255, 170}, {255, 255, 173}, {255, 255, 176}, {255, 255, 179}, {255, 255, 182}, {255, 255, 185}, {255, 255, 188}, {255, 255, 191}, {255, 255, 194}, {255, 255, 197}, {255, 255, 200}, {255, 255, 203}, {255, 255, 206}, {255, 255, 209}, {255, 255, 212}, {255, 255, 215}, {255, 255, 218}, {255, 255, 221}, {255, 255, 224}, {255, 255, 227}, {255, 255, 230}, {255, 255, 234}, {255, 255, 237}, {255, 255, 240}, {255, 255, 243}, {255, 255, 246}, {255, 255, 249}, {255, 255, 252}, {255, 255, 255}] ("Array 2") cluster{u8, u8, u8}[] [{0, 0, 0}, {2, 0, 0}, {3, 0, 0}, {5, 0, 0}, {7, 0, 0}, {9, 0, 0}, {11, 0, 0}, {13, 0, 3}, {15, 0, 3}, {17, 0, 3}, {19, 0, 3}, {21, 0, 3}, {23, 0, 3}, {25, 0, 3}, {27, 0, 3}, {27, 0, 7}, {31, 0, 7}, {33, 0, 7}, {35, 0, 7}, {37, 0, 7}, {39, 0, 7}, {41, 0, 7}, {43, 0, 7}, {45, 0, 7}, {47, 0, 11}, {49, 0, 11}, {51, 0, 11}, {53, 0, 11}, {55, 0, 11}, {57, 0, 11}, {59, 0, 11}, {59, 3, 11}, {63, 3, 11}, {65, 3, 11}, {67, 3, 11}, {69, 3, 11}, {71, 3, 15}, {73, 3, 15}, {75, 3, 15}, {79, 3, 15}, {81, 3, 15}, {83, 3, 15}, {85, 3, 15}, {87, 3, 15}, {87, 7, 15}, {91, 7, 15}, {93, 7, 15}, {95, 7, 15}, {97, 7, 15}, {99, 7, 15}, {101, 7, 15}, {103, 7, 15}, {105, 7, 15}, {107, 11, 15}, {109, 11, 15}, {111, 11, 15}, {113, 11, 15}, {115, 11, 15}, {117, 11, 15}, {119, 11, 15}, {123, 11, 15}, {125, 11, 15}, {127, 15, 15}, {129, 15, 15}, {131, 15, 19}, {133, 15, 19}, {135, 15, 19}, {137, 15, 19}, {139, 15, 19}, {139, 19, 19}, {143, 19, 19}, {145, 19, 19}, {147, 19, 19}, {149, 19, 19}, {151, 23, 19}, {153, 23, 19}, {155, 23, 19}, {156, 23, 19}, {157, 23, 19}, {159, 27, 19}, {161, 27, 19}, {163, 27, 19}, {165, 27, 19}, {166, 31, 19}, {167, 31, 19}, {169, 31, 19}, {171, 31, 19}, {171, 35, 19}, {175, 35, 19}, {176, 35, 19}, {177, 35, 19}, {179, 39, 19}, {180, 39, 19}, {181, 39, 19}, {183, 43, 19}, {185, 43, 19}, {187, 43, 19}, {187, 47, 19}, {189, 47, 19}, {191, 47, 19}, {191, 51, 19}, {192, 51, 19}, {191, 51, 19}, {195, 55, 19}, {195, 57, 19}, {195, 59, 19}, {199, 59, 19}, {199, 61, 19}, {199, 63, 19}, {201, 63, 19}, {203, 67, 19}, {204, 67, 19}, {205, 69, 19}, {207, 71, 19}, {207, 73, 19}, {207, 75, 19}, {207, 77, 19}, {209, 79, 19}, {211, 79, 19}, {211, 83, 19}, {211, 85, 19}, {211, 87, 19}, {213, 87, 19}, {215, 91, 19}, {215, 93, 19}, {215, 95, 19}, {215, 97, 19}, {217, 99, 19}, {219, 99, 19}, {219, 103, 19}, {219, 105, 19}, {219, 106, 19}, {219, 107, 19}, {219, 111, 19}, {221, 111, 19}, {223, 115, 19}, {223, 117, 23}, {223, 119, 23}, {223, 121, 23}, {223, 123, 23}, {223, 125, 23}, {225, 127, 23}, {227, 127, 23}, {227, 131, 23}, {227, 133, 27}, {227, 135, 27}, {227, 137, 27}, {227, 139, 27}, {227, 141, 29}, {229, 143, 31}, {231, 143, 31}, {231, 145, 31}, {231, 147, 31}, {231, 149, 31}, {231, 151, 35}, {231, 153, 35}, {231, 155, 35}, {233, 157, 35}, {235, 159, 37}, {235, 160, 39}, {235, 161, 39}, {235, 163, 39}, {235, 165, 43}, {235, 167, 43}, {235, 169, 45}, {235, 171, 47}, {235, 171, 47}, {237, 173, 47}, {239, 175, 49}, {239, 177, 51}, {239, 179, 51}, {239, 179, 53}, {239, 179, 55}, {239, 183, 59}, {239, 185, 59}, {239, 187, 61}, {239, 187, 63}, {239, 189, 65}, {241, 191, 67}, {243, 191, 69}, {243, 191, 71}, {243, 191, 73}, {243, 191, 75}, {243, 197, 75}, {243, 199, 79}, {243, 201, 81}, {243, 203, 83}, {243, 203, 85}, {243, 205, 87}, {243, 207, 87}, {243, 207, 91}, {245, 209, 93}, {247, 211, 95}, {247, 211, 97}, {247, 213, 99}, {247, 215, 103}, {247, 215, 105}, {247, 215, 107}, {247, 219, 107}, {247, 219, 111}, {247, 221, 113}, {247, 223, 115}, {247, 223, 119}, {247, 223, 121}, {247, 223, 123}, {247, 227, 123}, {247, 227, 127}, {247, 227, 129}, {247, 229, 131}, {247, 231, 135}, {249, 231, 135}, {251, 231, 139}, {251, 231, 143}, {251, 235, 143}, {251, 235, 147}, {251, 235, 149}, {251, 235, 151}, {251, 237, 153}, {251, 239, 155}, {251, 239, 159}, {251, 239, 161}, {251, 239, 163}, {251, 241, 167}, {251, 243, 167}, {251, 243, 171}, {251, 243, 173}, {251, 243, 175}, {251, 243, 179}, {251, 245, 181}, {251, 247, 183}, {251, 247, 187}, {251, 247, 189}, {251, 247, 191}, {251, 247, 193}, {251, 247, 195}, {251, 247, 199}, {251, 249, 201}, {251, 251, 203}, {251, 251, 207}, {251, 251, 209}, {251, 251, 211}, {251, 251, 213}, {251, 251, 215}, {251, 251, 219}, {251, 251, 221}, {251, 251, 223}, {251, 251, 227}, {251, 251, 229}, {251, 251, 231}, {251, 251, 235}, {251, 251, 237}, {251, 251, 239}, {251, 251, 243}, {251, 251, 245}, {251, 251, 247}, {251, 251, 251}] ("Array")] -> w310
              frame "Gray", Default {
              }
              frame "Red" {
              }
              frame "Green" {
              }
              frame "Blue" {
              }
              frame "Cyan" {
              }
              frame "Magenta" {
              }
              frame "Yellow" {
              }
              frame "Red-White" {
              }
              frame "Green-White" {
              }
              frame "Blue-White" {
              }
              frame "Fire" {
              }
              frame "Glow" {
              }
            }
            n176 = property class="ImageControl"(reference=w313, "Palette Type"=w311) -> (reference out=w312:refnum<vi>)  [unwired: 1 in, 1 out]
            n177 = property class="ImageControl"(reference=w323, "User Palette"=w310) -> ()  [unwired: 1 in, 2 out]
            n178 = property class="ImageControl"(reference=w312, "User Palette"=w310) -> ()  [unwired: 1 in, 2 out]
          }
          frame "Line Tool", "Pan Tool", "Point Tool", "Rectangle Tool", "Zoom Tool" {
            w344 = u32 0 items=["Zoom Tool"=8, "Selection Tool"=0, "Pan Tool"=9, "Point Tool"=1, "Line Tool"=2, "Rectangle Tool"=3, "Rotated Rectangle Tool"=12, "Polyline Tool"=10, "Polygon Tool"=5, "Freehand Tool"=11, "Closed Freehand Tool"=6, "Ellipse Tool"=4, "Annulus Tool"=7] ("Current ROI Tool")
            n179 = case shown="\"Point Tool\"" w341 {
              tunnel: [w348 w349 w350 w351 w352 w353] -> w340
              frame Default {
                w348 = u32 0 items=["Zoom Tool"=8, "Selection Tool"=0, "Pan Tool"=9, "Point Tool"=1, "Line Tool"=2, "Rectangle Tool"=3, "Rotated Rectangle Tool"=12, "Polyline Tool"=10, "Polygon Tool"=5, "Freehand Tool"=11, "Closed Freehand Tool"=6, "Ellipse Tool"=4, "Annulus Tool"=7] ("Current ROI Tool")
              }
              frame "Line Tool" {
                w349 = u32 2 items=["Zoom Tool"=8, "Selection Tool"=0, "Pan Tool"=9, "Point Tool"=1, "Line Tool"=2, "Rectangle Tool"=3, "Rotated Rectangle Tool"=12, "Polyline Tool"=10, "Polygon Tool"=5, "Freehand Tool"=11, "Closed Freehand Tool"=6, "Ellipse Tool"=4, "Annulus Tool"=7] ("Current ROI Tool")
              }
              frame "Pan Tool" {
                w350 = u32 9 items=["Zoom Tool"=8, "Selection Tool"=0, "Pan Tool"=9, "Point Tool"=1, "Line Tool"=2, "Rectangle Tool"=3, "Rotated Rectangle Tool"=12, "Polyline Tool"=10, "Polygon Tool"=5, "Freehand Tool"=11, "Closed Freehand Tool"=6, "Ellipse Tool"=4, "Annulus Tool"=7] ("Current ROI Tool")
              }
              frame "Point Tool" {
                w351 = u32 1 items=["Zoom Tool"=8, "Selection Tool"=0, "Pan Tool"=9, "Point Tool"=1, "Line Tool"=2, "Rectangle Tool"=3, "Rotated Rectangle Tool"=12, "Polyline Tool"=10, "Polygon Tool"=5, "Freehand Tool"=11, "Closed Freehand Tool"=6, "Ellipse Tool"=4, "Annulus Tool"=7] ("Current ROI Tool")
              }
              frame "Rectangle Tool" {
                w352 = u32 3 items=["Zoom Tool"=8, "Selection Tool"=0, "Pan Tool"=9, "Point Tool"=1, "Line Tool"=2, "Rectangle Tool"=3, "Rotated Rectangle Tool"=12, "Polyline Tool"=10, "Polygon Tool"=5, "Freehand Tool"=11, "Closed Freehand Tool"=6, "Ellipse Tool"=4, "Annulus Tool"=7] ("Current ROI Tool")
              }
              frame "Zoom Tool" {
                w353 = u32 8 items=["Zoom Tool"=8, "Selection Tool"=0, "Pan Tool"=9, "Point Tool"=1, "Line Tool"=2, "Rectangle Tool"=3, "Rotated Rectangle Tool"=12, "Polyline Tool"=10, "Polygon Tool"=5, "Freehand Tool"=11, "Closed Freehand Tool"=6, "Ellipse Tool"=4, "Annulus Tool"=7] ("Current ROI Tool")
              }
            }
            n180 = property class="ImageControl"(reference=w347) -> (reference out=w343:refnum<vi>, "Current ROI Tool"=w346:u32)  [unwired: 1 in, 1 out]
            n181 = Equal?(x=w346, y=w340) -> (x = y?=w345:bool)
            n182 = Select(t=w344, s=w345, f=w340) -> (s? t:f=w342:u32)
            n183 = property class="ImageControl"(reference=w343, "Current ROI Tool"=w342) -> ()  [unwired: 1 in, 2 out]
          }
          frame "Auto Scale Z" {
            w378 = u32 14 items=["Default"=10, "Most Significant Bits"=11, "Full Dynamic"=12, "Downshift"=13, "Given Range"=14, "90% Dynamic"=15, "Given Percent Range"=16] ("16-bit Display Mapping:Conversion Method")
            w377 = u32 10 items=["Default"=10, "Most Significant Bits"=11, "Full Dynamic"=12, "Downshift"=13, "Given Range"=14, "90% Dynamic"=15, "Given Percent Range"=16] ("16-bit Display Mapping:Conversion Method")
            n184 = for {
              tunnel: w375 -> [w383] mode=indexing
              tunnel: w372 -> [w384]
              tunnel: [w382] -> w373
              i -> [w382]
              stop <- w385 stop-if-true
              n185 = Equal?(x=w384, y=w383) -> (x = y?=w385:bool)
            }
            n186 = property class="ImageControl"(reference=w372) -> (reference out=w381:refnum<vi>, "16-bit Display Conversion Method"=w380:u32, "Value"=w362:variant)  [unwired: 1 in, 1 out]
            n187 = Index Array(array=w374, index=w373) -> (element=w371:refnum<vi>)
            n188 = property class="Clust (strict)"(reference=w371) -> ("Controls[]"=w370:refnum<vi>[])  [unwired: 1 in, 2 out]
            n189 = Variant To Data(type=T3 refnum ("New Image"), Variant=w362) -> (data=w360:T3)  [unwired: 1 in, 1 out]
            n190 = call "IMAQ Quantify 2"("Image"=w360) -> ("Global Report"=w361:T13)  [unwired: 8 in, 2 out]
            n191 = Equal?(x=w380, y=w377) -> (x = y?=w379:bool)
            n192 = Unbundle By Name(w361) -> ("Maximal Value"=w357:sgl, "Minimal Value"=w356:sgl)
            n193 = Select(t=w378, s=w379, f=w377) -> (s? t:f=w376:u32)
            n194 = To Long Integer(number=w357) -> (32bit integer=w359:i32)
            n195 = To Long Integer(number=w356) -> (32bit integer=w358:i32)
            n196 = To Single Precision Float(number=w357) -> (single precision float=w354:sgl)
            n197 = To Single Precision Float(number=w356) -> (single precision float=w355:sgl)
            n198 = property class="ImageControl"(reference=w381, "16-bit Display Conversion Method"=w376, "16-bit Display Maximum Value"=w359, "16-bit Display Minimum Value"=w358) -> ()  [unwired: 1 in, 2 out]
            n199 = Index Array(array=w370, index #1=2 ("index"), index #2=1 ("index")) -> (element #1=w367:refnum<vi>, element #2=w364:refnum<vi>)
            n200 = To Variant(anything=w354) -> (Variant=w366:variant)
            n201 = To Variant(anything=w355) -> (Variant=w365:variant)
            n202 = property class="Ctl"(reference=w367, "Value"=w366) -> ()  [unwired: 1 in, 2 out]
            n203 = property class="Ctl"(reference=w364, "Value"=w365) -> ()  [unwired: 1 in, 2 out]
          }
          frame "Auto Scale All" {
            n204 = for {
              tunnel: w386 -> [w388] mode=indexing
              w387 = u32 10 items=["Default"=10, "Most Significant Bits"=11, "Full Dynamic"=12, "Downshift"=13, "Given Range"=14, "90% Dynamic"=15, "Given Percent Range"=16] ("16-bit Display Mapping:Conversion Method")
              n205 = property class="ImageControl"(reference=w388, "16-bit Display Conversion Method"=w387) -> ()  [unwired: 1 in, 2 out]
            }
          }
          frame "Show Z Scale" {
            n206 = for {
              tunnel: w396 -> [w400] mode=indexing
              tunnel: w394 -> [w398]
              tunnel: [w397] -> w393
              i -> [w397]
              stop <- w399 stop-if-true
              n207 = Equal?(x=w398, y=w400) -> (x = y?=w399:bool)
            }
            n208 = Index Array(array=w395, index=w393) -> (element=w392:refnum<vi>)
            n209 = property class="Clust (strict)"(reference=w392) -> (reference out=w391:refnum<vi>, "Visible"=w390:bool)  [unwired: 1 in, 1 out]
            n210 = Not(x=w390) -> (.not. x?=w389:bool)
            n211 = property class="Clust (strict)"(reference=w391, "Visible"=w389) -> ()  [unwired: 1 in, 2 out]
          }
          frame "Show All Z Scale" {
            n212 = call "Lock Displays AE.vi"("Action"=Standard_Action."Read") -> ("Lock All Markers Out"=w408:bool, "Lock All AutoScale Out"=w404:bool, "Show All Z Scale Out"=w403:bool, "Lock Pan/Zoom Out"=w407:bool)  [unwired: 11 in]
            n213 = Not(x=w403) -> (.not. x?=w402:bool)
            n214 = call "Lock Displays AE.vi"("Lock All Markers"=w408, "Action"=Standard_Action."Write", "Lock All AutoScale"=w404, "Show All Z Scale"=w402, "Lock Pan/Zoom"=w407) -> ("Show All Z Scale Out"=w401:bool)  [unwired: 7 in, 3 out]
            n215 = for {
              tunnel: w409 -> [w414] mode=indexing
              tunnel: w401 -> [w413]
              n216 = Select(t=TRUE, s=w413, f=FALSE) -> (s? t:f=w410:bool)
              n217 = property class="Clust (strict)"(reference=w414, "Visible"=w410) -> ()  [unwired: 1 in, 2 out]
            }
          }
          frame "Lock All AutoScale" {
            n218 = call "Lock Displays AE.vi"("Action"=Standard_Action."Read") -> ("Lock All Markers Out"=w417:bool, "Lock All AutoScale Out"=w423:bool, "Show All Z Scale Out"=w415:bool, "Lock Pan/Zoom Out"=w416:bool)  [unwired: 11 in]
            n219 = Not(x=w423) -> (.not. x?=w424:bool)
            n220 = call "Lock Displays AE.vi"("Lock All Markers"=w417, "Action"=Standard_Action."Write", "Lock All AutoScale"=w424, "Show All Z Scale"=w415, "Lock Pan/Zoom"=w416) -> ("Lock All AutoScale Out"=w418:bool)  [unwired: 7 in, 3 out]
            n221 = for {
              tunnel: w420 -> [w433] mode=indexing
              tunnel: w419 -> [w432] mode=indexing
              tunnel: w418 -> [w425]
              w449 = u32 14 items=["Default"=10, "Most Significant Bits"=11, "Full Dynamic"=12, "Downshift"=13, "Given Range"=14, "90% Dynamic"=15, "Given Percent Range"=16] ("16-bit Display Mapping:Conversion Method")
              w448 = u32 10 items=["Default"=10, "Most Significant Bits"=11, "Full Dynamic"=12, "Downshift"=13, "Given Range"=14, "90% Dynamic"=15, "Given Percent Range"=16] ("16-bit Display Mapping:Conversion Method")
              n222 = property class="ImageControl" props=["16-bit Display Conversion Method", "Value"](reference=w433) -> (reference out=w450:refnum<vi>, "Value"=w426:variant)  [unwired: 1 in, 2 out]
              n223 = property class="Clust (strict)"(reference=w432) -> ("Controls[]"=w446:refnum<vi>[])  [unwired: 1 in, 2 out]
              n224 = Variant To Data(type="", Variant=w426) -> (data=w429:string)  [unwired: 1 in, 1 out]
              n225 = Not Equal?(x=w429, y="") -> (x != y?=w427:bool)
              n226 = case shown="True" w427 {
                tunnel: [T13 {"Mean Value"=0.0, "Standard Variation"=0.0, "Minimal Value"=0.0, "Maximal Value"=0.0, "Area (calibrated)"=0.0, "Area (pixels)"=0, "%"=0.0, "Calibration Valid"=FALSE} ("Global Report") w455] -> w431
                tunnel: w426 -> [_ w452]
                frame False {
                }
                frame True {
                  n227 = Variant To Data(type=T3 refnum ("New Image"), Variant=w452) -> (data=w454:T3)  [unwired: 1 in, 1 out]
                  n228 = call "IMAQ Quantify 2"("Image"=w454) -> ("Global Report"=w455:T13)  [unwired: 8 in, 2 out]
                }
              }
              n229 = Unbundle By Name(w431) -> ("Maximal Value"=w437:sgl, "Minimal Value"=w436:sgl)
              n230 = Select(t=w449, s=w425, f=w448) -> (s? t:f=w447:u32)
              n231 = To Long Integer(number=w437) -> (32bit integer=w439:i32)
              n232 = To Long Integer(number=w436) -> (32bit integer=w438:i32)
              n233 = To Single Precision Float(number=w437) -> (single precision float=w434:sgl)
              n234 = To Single Precision Float(number=w436) -> (single precision float=w435:sgl)
              n235 = Index Array(array=w446, index #1=2 ("index"), index #2=1 ("index")) -> (element #1=w443:refnum<vi>, element #2=w440:refnum<vi>)
              n236 = property class="ImageControl"(reference=w450, "16-bit Display Conversion Method"=w447, "16-bit Display Maximum Value"=w439, "16-bit Display Minimum Value"=w438) -> ()  [unwired: 1 in, 2 out]
              n237 = To Variant(anything=w434) -> (Variant=w442:variant)
              n238 = To Variant(anything=w435) -> (Variant=w441:variant)
              n239 = property class="Ctl"(reference=w443, "Value"=w442) -> ()  [unwired: 1 in, 2 out]
              n240 = property class="Ctl"(reference=w440, "Value"=w441) -> ()  [unwired: 1 in, 2 out]
            }
          }
          frame "Lock All Markers" {
            n241 = property class="ImageControl"(reference=w458) -> ("ROI"=w459:T12)  [unwired: 1 in, 2 out]
            n242 = call "Lock Displays AE.vi"("Action"=Standard_Action."Read") -> ("Lock All Markers Out"=w463:bool, "Lock All AutoScale Out"=w460:bool, "Show All Z Scale Out"=w456:bool, "Lock Pan/Zoom Out"=w465:bool)  [unwired: 11 in]
            n243 = Not(x=w463) -> (.not. x?=w464:bool)
            n244 = call "Lock Displays AE.vi"("Lock All Markers"=w464, "Action"=Standard_Action."Write", "Lock All AutoScale"=w460, "Show All Z Scale"=w456, "Lock Pan/Zoom"=w465) -> ()  [unwired: 7 in, 4 out]
            n245 = for {
              tunnel: w457 -> [w467] mode=indexing
              tunnel: w459 -> [w466]
              n246 = property class="ImageControl"(reference=w467, "ROI"=w466) -> ()  [unwired: 1 in, 2 out]
            }
          }
          frame "Lock Zoom/Pan" {
            n247 = property class="ImageControl"(reference=w469) -> ("ZoomSingle"=w472:cluster{"X":sgl, "Y":sgl}, "Image Center Position"=w471:cluster{"X":u32, "Y":u32})  [unwired: 1 in, 2 out]
            n248 = call "Lock Displays AE.vi"("Action"=Standard_Action."Read") -> ("Lock All Markers Out"=w476:bool, "Lock All AutoScale Out"=w475:bool, "Show All Z Scale Out"=w468:bool, "Lock Pan/Zoom Out"=w473:bool)  [unwired: 11 in]
            n249 = Not(x=w473) -> (.not. x?=w474:bool)
            n250 = call "Lock Displays AE.vi"("Lock All Markers"=w476, "Action"=Standard_Action."Write", "Lock All AutoScale"=w475, "Show All Z Scale"=w468, "Lock Pan/Zoom"=w474) -> ()  [unwired: 7 in, 4 out]
            n251 = for {
              tunnel: w470 -> [w481] mode=indexing
              tunnel: w472 -> [w480]
              tunnel: w471 -> [w479]
              n252 = property class="ImageControl"(reference=w481, "ZoomSingle"=w480, "Image Center Position"=w479) -> ()  [unwired: 1 in, 2 out]
            }
          }
          frame "Clear All Markers", "Clear Markers" {
            n253 = Build Array(w486) -> (w485:refnum<vi>[])
            n254 = Equal?(x="Clear Markers", y=w488) -> (x = y?=w483:bool)
            n255 = Select(t=w485, s=w483, f=w484) -> (s? t:f=w482:refnum<vi>[])
            n256 = for {
              tunnel: w482 -> [w489] mode=indexing
              n257 = property class="ImageControl"(reference=w489, "ROI"=T12 {"Global Rectangle"=[], "Contours"=[]}) -> ("Value"=w490:variant)  [unwired: 1 in, 2 out]
              n258 = Variant To Data(type=T3 refnum ("New Image"), Variant=w490) -> (data=w493:T3)  [unwired: 1 in, 1 out]
              n259 = Not A Number/Path/Refnum?(number/path/refnum=w493) -> (NaN/Path/Refnum?=w492:bool)
              n260 = case shown="False" w492 {
                tunnel: w493 -> [w501 _]
                frame False {
                  w495 = "Image ROI" ("element")
                  n261 = call "IMAQ Clear Overlay"("Image"=w501) -> ("Image Out"=w500:T3)  [unwired: 9 in, 1 out]
                  n262 = call "IMAQ Get Custom Keys"("Image"=w500) -> ("Keys"=w499:string[], "Image (duplicate)"=w496:T3)  [unwired: 7 in, 2 out]
                  n263 = Search 1D Array(1D array=w499, element=w495) -> (index of element=w498:i32)  [unwired: 1 in]
                  n264 = Less Than 0?(x=w498) -> (x < 0?=w497:bool)
                  n265 = case shown="False" w497 {
                    tunnel: w496 -> [w503 _]
                    tunnel: w495 -> [w502 _]
                    frame False {
                      n266 = call "IMAQ Remove Custom Data"("Key"=w502, "Image"=w503) -> ()  [unwired: 7 in, 3 out]
                    }
                    frame True {
                    }
                  }
                }
                frame True {
                }
              }
            }
          }
          frame "Reset Zoom" {
            n267 = call "Lock Displays AE.vi"("Action"=Standard_Action."Read") -> ("Lock Pan/Zoom Out"=w508:bool)  [unwired: 11 in, 3 out]
            n268 = Build Array(w510) -> (w505:refnum<vi>[])
            n269 = Not(x=w508) -> (.not. x?=w507:bool)
            n270 = Select(t=w505, s=w507, f=w506) -> (s? t:f=w504:refnum<vi>[])
            n271 = for {
              tunnel: w504 -> [w514] mode=indexing
              w511 = u32 0 items=["Zoom Tool"=8, "Selection Tool"=0, "Pan Tool"=9, "Point Tool"=1, "Line Tool"=2, "Rectangle Tool"=3, "Rotated Rectangle Tool"=12, "Polyline Tool"=10, "Polygon Tool"=5, "Freehand Tool"=11, "Closed Freehand Tool"=6, "Ellipse Tool"=4, "Annulus Tool"=7] ("Current ROI Tool")
              n272 = property class="ImageControl"(reference=w514, "Zoom to Fit Mode"=TRUE) -> (reference out=w512:refnum<vi>)  [unwired: 1 in, 1 out]
              n273 = property class="ImageControl"(reference=w512, "Current ROI Tool"=w511) -> ()  [unwired: 1 in, 2 out]
            }
          }
          frame "Merge Tool" {
            n274 = control-ref of="This VI"() -> (w515:refnum<vi>)
            n275 = call "Display Module - Run Merge Tool.vi"("Calling VI Ref"=w515) -> ()  [unwired: 15 in]
          }
          frame "Load Image" {
          }
          frame "Save Image" {
            n276 = property class="ImageControl"(reference=w519) -> ("Value"=w518:variant)  [unwired: 1 in, 2 out]
            n277 = Variant To Data(type=T3 refnum ("Image"), Variant=w518) -> (data=w516:T3)  [unwired: 1 in, 1 out]
            n278 = call "File Dialog"("prompt"="Save TIF Image", "button label"="Save", "pattern (all files)"="*.tif", "pattern label"="TIF") -> ("selected path"=w520:path, "error out"=w521:errorcluster)  [unwired: 8 in, 2 out]
            n279 = case shown="No Error" w521 {
              tunnel: w520 -> [w544 _]
              tunnel: w516 -> [w545 _]
              frame No Error {
                w528 = 0.0 ("Z Step (µm)")
                w529 = u32 1 ("No. of Frames")
                w530 = 1.0 ("Pixel Height (µm)")
                n280 = call "IMAQ ImageToArray"("Image"=w545) -> ("Image Pixels (U16)"=w527:u16[][])  [unwired: 3 in, 4 out]
                n281 = Array Size(array=w527) -> (size(s)=w536:i32[])
                n282 = To Unsigned Long Integer(number=w536) -> (unsigned 32bit integer=w526:u32[])
                n283 = Index Array(array=w526, index #1=1 ("index"), index #2=0 ("index")) -> (element #1=w533:u32, element #2=w532:u32)
                n284 = Bundle By Name(cluster=T14 {"Image Width (Pixels)"=0, "Image Height (Pixels)"=0, "Pixel Width (µm)"=0.0, "Pixel Height (µm)"=0.0, "Bits Per Sample (e.g. 16)"=0, "No. of Frames"=0, "No. of Slices"=0, "Time Step (sec)"=0.0, "Z Step (µm)"=0.0} ("Image Info"), "Image Width (Pixels)"=w533, "Image Height (Pixels)"=w532, "Pixel Width (µm)"=w530, "Pixel Height (µm)"=w530, "Bits Per Sample (e.g. 16)"=u32 16, "No. of Frames"=w529, "No. of Slices"=w529, "Time Step (sec)"=w528, "Z Step (µm)"=w528) -> (w537:T14)
                n285 = call "Write TIFF Header.vi"("File Path"=w544, "Image Info"=w537) -> ("File Ref"=w543:refnum<file>, "Byte Order"=w539:T17, "Error"=w540:errorcluster)  [unwired: 11 in]
                n286 = Write to Binary File(file (use dialog)=w543, data=w527, error in=w540, 9:w539) -> (refnum out=w542:refnum<file>, error out=w541:errorcluster)  [unwired: 2 in, 1 out]
                n287 = Close File(refnum=w542, error in=w541) -> ()  [unwired: 2 out]
              }
              frame Error {
              }
            }
          }
        }
      }
      event "Channel 1", "Channel 2", "Channel 3", "Channel 4", "Channel 5", "Channel 6": Mouse Up {
        # "1: Left Click\n2: Right Click\n3: Middle Click"
        n288 = event-data() -> ("CtlRef"=w547:refnum<vi>)  [unwired: 1 in, 1 out]
        n289 = property class="ImageControl"(reference=w547) -> ("ZoomSingle"=w555:cluster{"X":sgl, "Y":sgl}, "Image Center Position"=w551:cluster{"X":u32, "Y":u32})  [unwired: 1 in, 2 out]
        n290 = property class="ImageControl" props=["ROI", "Value"](reference=w547) -> ("ROI"=w548:T12)  [unwired: 1 in, 3 out]
        n291 = call "Lock Displays AE.vi"("Action"=Standard_Action."Read") -> ("Lock Pan/Zoom Out"=w552:bool)  [unwired: 11 in, 3 out]
        n292 = call "Lock Displays AE.vi"("Action"=Standard_Action."Read") -> ("Lock All Markers Out"=w556:bool)  [unwired: 11 in, 3 out]
        n293 = case shown="True" w552 {
          tunnel: w553 -> [_ w568]
          tunnel: w555 -> [_ w567]
          tunnel: w551 -> [_ w566]
          frame False {
          }
          frame True {
            n294 = for {
              tunnel: w568 -> [w571] mode=indexing
              tunnel: w567 -> [w570]
              tunnel: w566 -> [w569]
              n295 = property class="ImageControl"(reference=w571, "ZoomSingle"=w570, "Image Center Position"=w569) -> ()  [unwired: 1 in, 2 out]
            }
          }
        }
        n296 = case shown="True" w556 {
          tunnel: w553 -> [_ w573]
          tunnel: w548 -> [_ w572]
          frame False {
          }
          frame True {
            n297 = for {
              tunnel: w573 -> [w575] mode=indexing
              tunnel: w572 -> [w574]
              n298 = property class="ImageControl"(reference=w575, "ROI"=w574) -> ()  [unwired: 1 in, 2 out]
            }
          }
        }
        n299 = Unbundle By Name(w548) -> ("Contours"=w550:T18)
        n300 = Array Size(array=w550) -> (size(s)=w546:i32)
        n301 = Equal To 0?(x=w546) -> (x = 0?=w549:bool)
        n302 = case shown="False" w549 {
          tunnel: w548 -> [w565 _]
          tunnel: w547 -> [w564 _]
          frame False {
            n303 = property class="ImageControl"(reference=w564) -> ("Value"=w561:variant)  [unwired: 1 in, 2 out]
            n304 = Flatten To JSON(anything=w565) -> (JSON string=w562:string)  [unwired: 2 in, 1 out]
            n305 = Variant To Data(type=T3 refnum ("New Image"), Variant=w561) -> (data=w559:T3)  [unwired: 1 in, 1 out]
            n306 = call "IMAQ Write Custom Data"("Custom Data In"=w562, "Key"="Image ROI", "Image"=w559) -> ()  [unwired: 7 in, 2 out]
          }
          frame True {
          }
        }
      }
      event "Channel 1", "Channel 2", "Channel 3", "Channel 4", "Channel 6", "Channel 5": Mouse Enter; "Channel 1", "Channel 2", "Channel 3", "Channel 4", "Channel 5", "Channel 6": Mouse Leave {
        w576 = Standard_Action."Write" ("Action")
        n307 = event-data() -> ("Type"=w579:T11, "CtlRef"=w578:refnum<vi>)  [unwired: 1 in]
        n308 = call "Current Display Mouse.vi"("Event Type"=w579, "Action"=w576, "IMAQ Image Display Ref"=w578) -> ()  [unwired: 11 in, 2 out]
        n309 = call "Main Info Bar Message AE.vi"("Action"=w576, "Message"="") -> ()  [unwired: 13 in, 1 out]
      }
      event Value Change {
        w586 = u32 14 items=["Default"=10, "Most Significant Bits"=11, "Full Dynamic"=12, "Downshift"=13, "Given Range"=14, "90% Dynamic"=15, "Given Percent Range"=16] ("16-bit Display Mapping:Conversion Method")
        n310 = event-data() -> ("NewVal.Z Scale Max"=w583:sgl, "NewVal.Z Scale Min"=w584:sgl, "CtlRef"=w585:refnum<vi>)  [unwired: 1 in]
        n311 = for {
          tunnel: w590 -> [w592] mode=indexing
          tunnel: [w594] -> w588
          tunnel: w585 -> [w593]
          i -> [w594]
          stop <- w595 stop-if-true
          n312 = Equal?(x=w593, y=w592) -> (x = y?=w595:bool)
        }
        n313 = To Long Integer(number=w583) -> (32bit integer=w582:i32)
        n314 = To Long Integer(number=w584) -> (32bit integer=w581:i32)
        n315 = Index Array(array=w589, index=w588) -> (element=w587:refnum<vi>)
        n316 = property class="ImageControl"(reference=w587, "16-bit Display Maximum Value"=w582, "16-bit Display Minimum Value"=w581, "16-bit Display Conversion Method"=w586) -> ()  [unwired: 1 in, 2 out]
      }
      event Key Down; Key Up {
        # "Switch to the Pan Tool when the space bar is held down"
        n317 = event-data() -> ("Type"=w602:T11, "ScanCode"=w600:i16)  [unwired: 1 in]
        n318 = Equal?(x=lveventtype."Key Down", y=w602) -> (x = y?=w596:bool)
        n319 = Equal?(x=w600, y=i16 57) -> (x = y?=w598:bool)
        n320 = case shown="True" w598 {
          tunnel: w597 -> [_ w608]
          tunnel: w596 -> [_ w607]
          frame False {
          }
          frame True {
            w605 = u32 0 items=["Zoom Tool"=8, "Selection Tool"=0, "Pan Tool"=9, "Point Tool"=1, "Line Tool"=2, "Rectangle Tool"=3, "Rotated Rectangle Tool"=12, "Polyline Tool"=10, "Polygon Tool"=5, "Freehand Tool"=11, "Closed Freehand Tool"=6, "Ellipse Tool"=4, "Annulus Tool"=7] ("Current ROI Tool")
            w606 = u32 9 items=["Zoom Tool"=8, "Selection Tool"=0, "Pan Tool"=9, "Point Tool"=1, "Line Tool"=2, "Rectangle Tool"=3, "Rotated Rectangle Tool"=12, "Polyline Tool"=10, "Polygon Tool"=5, "Freehand Tool"=11, "Closed Freehand Tool"=6, "Ellipse Tool"=4, "Annulus Tool"=7] ("Current ROI Tool")
            n321 = Select(t=w606, s=w607, f=w605) -> (s? t:f=w604:u32)
            n322 = for {
              tunnel: w608 -> [w610] mode=indexing
              tunnel: w604 -> [w609]
              n323 = property class="ImageControl"(reference=w610, "Current ROI Tool"=w609) -> ()  [unwired: 1 in, 2 out]
            }
          }
        }
      }
      event "Settings": Value Change {
        n324 = event-data() -> ("NewVal"=w611:bool, "CtlRef"=w612:refnum<vi>)  [unwired: 1 in]
        n325 = case shown="True" w611 {
          tunnel: w612 -> [_ w623]
          frame False {
            n326 = property on="Settings Menu" class="Clust (strict)"("Visible"=FALSE, "Left"=-100 ("Position:Left"), "Top"=0 ("Position:Top")) -> ()  [unwired: 2 in, 2 out]
          }
          frame True {
            n327 = property class="Bool (strict)"(reference=w623) -> ("Left"=w622:i32, "Top"=w617:i32)  [unwired: 1 in, 2 out]
            n328 = property on="Settings Menu" class="Clust (strict)"() -> ("Height"=w620:u32)  [unwired: 2 in, 2 out]
            n329 = To Long Integer(number=w620) -> (32bit integer=w618:i32)
            n330 = Subtract(x=w617, y=w618) -> (x-y=w619:i32)
            n331 = property on="Settings Menu" class="Clust (strict)"("Visible"=TRUE, "Left"=w622, "Top"=w619) -> ()  [unwired: 2 in, 2 out]
          }
        }
      }
      event "Settings Menu": Value Change {
        # "0: Refresh Rate\n1: Display Order\n2: Display On / Off"
        n332 = event-data() -> ("NewVal"=w630:T1)  [unwired: 1 in]
        n333 = local write "Settings"(FALSE ("Settings")) -> ()
        n334 = Cluster To Array(cluster=w630) -> (array=w629:bool[])
        n335 = property on="Settings Menu" class="Clust (strict)"("Visible"=FALSE, "Left"=-100 ("Position:Left"), "Top"=0 ("Position:Top"), "Value"=T1 {"Refresh Rate"=FALSE, "Change Display Order"=FALSE, "Display On / Off"=FALSE} ("Settings Menu")) -> ()  [unwired: 2 in, 2 out]
        n336 = Search 1D Array(1D array=w629, element=TRUE, start index (0)=0) -> (index of element=w626:i32)
        n337 = case shown="2" w626 {
          tunnel: w625 -> [_ _ w646 w656]
          tunnel: w624 -> [_ _ w639 w649]
          frame Default {
          }
          frame 0 {
            n338 = local read "Refresh Rate (ms)"() -> (w638:u32)
            n339 = call "Display Module Refresh Rate.vi"("Refresh Rate In"=w638) -> ("Refresh Rate Out"=w637:u32)  [unwired: 14 in]
            n340 = local write "Refresh Rate (ms)"(w637) -> ()
          }
          frame 1 {
            n341 = vi-ref "Display Module - Set Display Order.vi"() -> (w645:refnum<vi>)
            n342 = Get Notifier Status(notifier=w646) -> (current notification=w640:T3[])  [unwired: 1 in, 4 out]
            n343 = property class="VI Interface Type 0"(reference=w645) -> ("Path"=w644:path)  [unwired: 1 in, 2 out]
            n344 = Open VI Reference(type specifier VI Refnum (for type only)=w645, vi path=w644, options=128) -> (vi reference=w643:refnum<vi>)  [unwired: 3 in, 1 out]
            n345 = call-by-ref "Start Asynchronous Call"(reference=w643, "Image Refs"=w640, "IMAQ Display Refs"=w639) -> (reference out=w642:refnum<vi>)  [unwired: 15 in, 1 out]
            n346 = Close Reference(reference=w642) -> ()  [unwired: 1 in, 1 out]
          }
          frame 2 {
            n347 = Get Notifier Status(notifier=w656) -> (notifier out=w654:refnum<notifier>, current notification=w655:T3[])  [unwired: 1 in, 3 out]
            n348 = call "Display Module - All Images Active.vi"("Image Refs In"=w655) -> ("Image Refs Out"=w650:T3[])  [unwired: 14 in]
            n349 = vi-ref "Display Module - Switch On and Off.vi"() -> (w653:refnum<vi>)
            n350 = Send Notification(notification=w650, notifier=w654) -> ()  [unwired: 1 in, 2 out]
            n351 = property class="VI Interface Type 1"(reference=w653) -> ("Path"=w652:path)  [unwired: 1 in, 2 out]
            n352 = Open VI Reference(type specifier VI Refnum (for type only)=w653, vi path=w652, options=128) -> (vi reference=w651:refnum<vi>)  [unwired: 3 in, 1 out]
            n353 = call-by-ref "Start Asynchronous Call"(reference=w651, "Image Refs"=w650, "IMAQ Display Refs"=w649) -> (reference out=w648:refnum<vi>)  [unwired: 15 in, 1 out]
            n354 = Close Reference(reference=w648) -> ()  [unwired: 1 in, 1 out]
          }
        }
      }
      event "lock scale": Value Change {
        n355 = event-data() -> ()  [unwired: 1 in, 1 out]
        n356 = for {
          tunnel: w659 -> [w666] mode=indexing
          tunnel: w658 -> [w667] mode=indexing
          w663 = sgl 50.0 ("single precision float")
          w664 = sgl 200.0 ("single precision float")
          w665 = u32 14 items=["Default"=10, "Most Significant Bits"=11, "Full Dynamic"=12, "Downshift"=13, "Given Range"=14, "90% Dynamic"=15, "Given Percent Range"=16] ("16-bit Display Mapping:Conversion Method")
          n357 = property class="Clust (strict)"(reference=w667) -> ("Controls[]"=w675:refnum<vi>[])  [unwired: 1 in, 2 out]
          n358 = To Long Integer(number=w664) -> (32bit integer=w661:i32)
          n359 = To Long Integer(number=w663) -> (32bit integer=w660:i32)
          n360 = To Single Precision Float(number=w664) -> (single precision float=w662:sgl)
          n361 = To Single Precision Float(number=w663) -> (single precision float=w668:sgl)
          n362 = Index Array(array=w675, index #1=2 ("index"), index #2=1 ("index")) -> (element #1=w672:refnum<vi>, element #2=w669:refnum<vi>)
          n363 = To Variant(anything=w662) -> (Variant=w671:variant)
          n364 = To Variant(anything=w668) -> (Variant=w670:variant)
          n365 = property class="Ctl"(reference=w672, "Value"=w671) -> ()  [unwired: 1 in, 2 out]
          n366 = property class="Ctl"(reference=w669, "Value"=w670) -> ()  [unwired: 1 in, 2 out]
          n367 = local write "Max"(w661) -> ()
          n368 = local write "Min"(w660) -> ()
          n369 = property class="ImageControl"(reference=w666, "16-bit Display Conversion Method"=w665, "16-bit Display Maximum Value"=w661, "16-bit Display Minimum Value"=w660) -> ()  [unwired: 1 in, 2 out]
        }
      }
      event "Min", "Max": Value Change {
        n370 = event-data() -> ()  [unwired: 1 in, 6 out]
        n371 = for {
          tunnel: w678 -> [w683] mode=indexing
          tunnel: w677 -> [w684] mode=indexing
          w682 = u32 14 items=["Default"=10, "Most Significant Bits"=11, "Full Dynamic"=12, "Downshift"=13, "Given Range"=14, "90% Dynamic"=15, "Given Percent Range"=16] ("16-bit Display Mapping:Conversion Method")
          n372 = property class="Clust (strict)"(reference=w684) -> ("Controls[]"=w692:refnum<vi>[])  [unwired: 1 in, 2 out]
          n373 = To Single Precision Float(number="Max") -> (single precision float=w681:sgl)
          n374 = To Single Precision Float(number="Min") -> (single precision float=w685:sgl)
          n375 = Index Array(array=w692, index #1=2 ("index"), index #2=1 ("index")) -> (element #1=w689:refnum<vi>, element #2=w686:refnum<vi>)
          n376 = To Variant(anything=w681) -> (Variant=w688:variant)
          n377 = To Variant(anything=w685) -> (Variant=w687:variant)
          n378 = property class="Ctl"(reference=w689, "Value"=w688) -> ()  [unwired: 1 in, 2 out]
          n379 = property class="Ctl"(reference=w686, "Value"=w687) -> ()  [unwired: 1 in, 2 out]
          n380 = property class="ImageControl"(reference=w683, "16-bit Display Conversion Method"=w682, "16-bit Display Maximum Value"="Max", "16-bit Display Minimum Value"="Min") -> ()  [unwired: 1 in, 2 out]
        }
      }
      event "Exit": Value Change {
        n381 = event-data() -> ("NewVal"=w697:bool)  [unwired: 1 in]
        n382 = Close Reference(reference=w696) -> ()  [unwired: 1 in, 1 out]
        n383 = call "IMAQ Dispose"("Image"=w695) -> ()  [unwired: 5 in, 1 out]
        n384 = call "Main Info Bar Message AE.vi"("Action"=Standard_Action."Write", "Message"="") -> ()  [unwired: 13 in, 1 out]
      }
    }
  }
